vi "VIH UI - Property Page - Master Rule.vi"() -> ()   [LabVIEW 2014]
doc: "::: VI Helpeks :::\nCopyright (c) 2000-2026 Konstantin Shifershteyn. All rights reserved."
uses:
  _VIH HelpGen.llb/VIH HelpGen Typedef - Enum - Default,Enable,Disable.ctl
  _VIH HelpGen.llb/VIH HelpGen Typedef - Enum - Description Mode.ctl
  _VIH UI Controls.llb/VIH UI Control - Button - Insert HREF.ctl
  _VIH UI Controls.llb/VIH UI Control - Button - Insert Bold.ctl
  _VIH UI Controls.llb/VIH UI Control - Button - Insert Italic.ctl
  _VIH UI Controls.llb/VIH UI Control - Button - Insert Underline.ctl
  _VIH Project Manager.llb/VIH Project Tree Typedef - Tree Refnum.ctl
  VIH UI Typedef - Property Page ExtCommand.ctl
  <vilib>/Utility/miscctls.llb/LVPositionTypeDef.ctl
  <vilib>/Utility/miscctls.llb/LVPointTypeDef.ctl
  <vilib>/Utility/miscctls.llb/LVRowAndColumnUnsignedTypeDef.ctl
  <vilib>/Utility/miscctls.llb/LVSelectionTypeDef.ctl
  _VIH Support Library.llb/VIH Utility - APP - Is Value Changed (STR).vi
panel:
  out "CategoryTitle":string
  in  "%UPDATE":bool
  in  "%STOP":bool
  in  "Category List":i32(listbox)
  in  "TreeRef":T1
  in  "Tab Control":enum32{"0", "1", "2", "3", "4", "5", "6", "7"}(tab) caption="Master Rule"
  in  "PI_AddInfo":string caption="Additional Information"
  in  "PI_Email":string caption="Contact E-mail"
  in  "PI_Website":string caption="Web site"
  in  "PI_Version":string caption="Version"
  in  "PI_Copyright":string caption="Legal Copyright"
  in  "PI_Company":string caption="Company Name"
  in  "PI_Author":string caption="Author Name"
  in  "PI_Product":string caption="Product Name"
  in  "ProductInfoText":string caption="Product Info section"
  in  "ProductInfoMode":T2 caption="Product Info mode"
  out "Group Name":string
  in  "Comments":string
  in  "Dst_Image Dir":path caption="Subfolder to save image files"
  in  "Dst_HTML Dir":path caption="Subfolder to save HTML files"
  in  "Dst_JS Dir":path caption="Subfolder to save JavaScript files"
  in  "Dst_CSS Dir":path caption="Subfolder to save CSS files"
  in  "Build Root Dir":path caption="Build Root Folder"
  in  "Src_VI Template":path caption="VI Help Template File"
  in  "Src_Menu Template":path caption="Menu Help Template File"
  in  "Src_PolyVI Template":path caption="Polymorphic VI Help Template File"
  out "JS File":path caption="JS File Path"
  in  "JS List":i32[](listbox) caption="JavaScript Files"
  in  "%JS List_Add":bool caption="Add JavaScript File"
  in  "%JS List_Remove":bool caption="Remove JavaScript File"
  out "CSS File":path caption="CSS File Path"
  in  "CSS List":i32[](listbox) caption="CSS Files"
  in  "%CSS List_Add":bool caption="Add CSS File"
  in  "%CSS List_Remove":bool caption="Remove CSS File"
  in  "VIDetailsMode":T3 caption="Default VI details mode"
  in  "PVIIDscrMode":T3 caption="Default Polymorphic VI Instance description mode"
  in  "MenuItemIcons":T2 caption="Generate Palette Item Icons"
  in  "MenuDscrMode":T3 caption="Default Palette description mode"
  in  "VIDscrMode":T3 caption="Default VI description mode"
  in  "Ctl_EnumValues":T2 caption="Build list of Enum and Ring values"
  in  "Ctl_ClustMembers":T2 caption="Expand cluster members"
  in  "Ctl_DscrMode":T3 caption="VI Controls/Terminals description mode"
  in  "%CtrlRule_Insert_<I>":T4 caption="Format as Italic"
  in  "%CtrlRule_Insert_<U>":T5 caption="Format as Underline"
  in  "%CtrlRule_Insert_<B>":T6 caption="Format as Bold"
  in  "%CtrlRule_Insert_HREF":T7 caption="Insert Reference"
  in  "CtrlRule_Description":string caption="Description"
  in  "CtrlRule_CustomName":string caption="Custom Control Name"
  in  "CtrlRule_DscrMode":T3 caption="Description mode"
  in  "CtrlRule_CustomRule":bool caption="Enable custom rule"
  in  "CtrlRule_CtrlID":string caption="Control Identifier"
  in  "%CtrlRule_Edit_Enum":bool caption="Edit Enumerated Values Description"
  in  "CtrlRule_EnumValues":T2 caption="Enum and Ring values"
  in  "CtrlRule_ClustMembers":T2 caption="Cluster members"
  in  "%CtrlRule_Copy":bool caption="Copy"
  in  "%CtrlRule_Paste":bool caption="Paste"
  in  "%CtrlRule_Import":bool caption="Import VI Terminal Controls"
  in  "CtrlRule List":i32[](listbox)
  in  "%CtrlRule_Remove":bool caption="Remove"
  in  "%CtrlRule_Add":bool caption="Add"
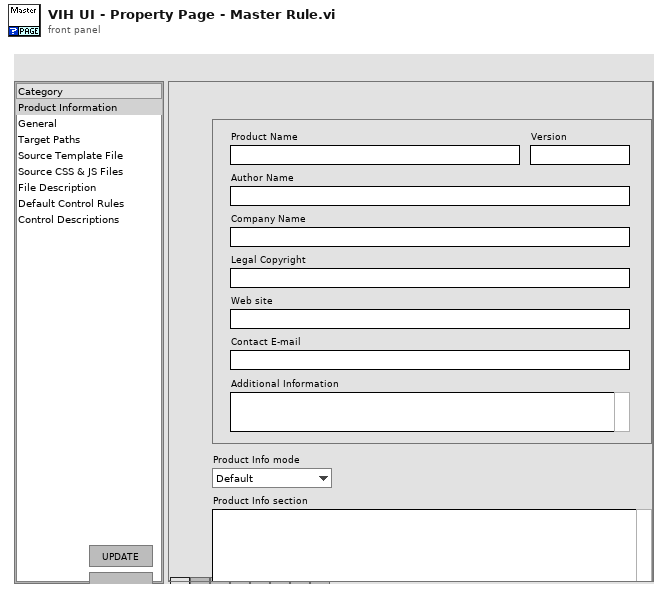
[diagram p1: front panel]
types:
  T1 = typedef "VIH Project Tree Typedef - Tree Refnum.ctl" = refnum<vi>
  T2 = typedef "VIH HelpGen Typedef - Enum - Default,Enable,Disable.ctl" = enum16{"Default", "Enable", "Disable"}
  T3 = typedef "VIH HelpGen Typedef - Enum - Description Mode.ctl" = enum16{"Default", "Description", "Description1", "Description2", "Custom", "None"}
  T4 = typedef "VIH UI Control - Button - Insert Italic.ctl" = bool
  T5 = typedef "VIH UI Control - Button - Insert Underline.ctl" = bool
  T6 = typedef "VIH UI Control - Button - Insert Bold.ctl" = bool
  T7 = typedef "VIH UI Control - Button - Insert HREF.ctl" = bool
  T8 = typedef "VIH UI Typedef - Property Page ExtCommand.ctl" = cluster{"Action":string, "Project Tree":T1, "Params":string[]}
  T9 = enum16{"Open", "Close", "Update", "Set Category"}
  T10 = enum32{"Invalid", "Standard", "Closed", "Hidden", "Minimized", "Maximized"}
  T11 = enum8{"Enabled", "Disabled", "Disabled and Grayed Out"}
  T12 = typedef "LVSelectionTypeDef.ctl" = cluster{"Selection Start":u32, "Selection End":u32}
  T13 = typedef "eventvkey.ctl" = enum16{"ASCII", "Enter", "Return", "Shift", "Ctrl", "Alt", "Cmd", "Opt", "Caps", "NumLock", "Clear", "Break", "Up", "Down", "Left", "Right", "Insert", "Delete", "Home", "End", "PageUp", "PageDown", "Escape", "Help", "Pause", "ScrollLock", "F1", "F2", "F3", "F4", "F5", "F6", "F7", "F8", "F9", "F10", "F11", "F12", "F13", "F14", "F15", "F16", "F17", "F18", "F19", "F20", "F21", "F22", "F23", "F24", "Play", "VolumeUp", "VolumeDown", "Mute", "Two Byte Char"}
  T14 = cluster{"Shift":bool, "Ctrl":bool, "Alt":bool, "Cmd":bool, "Opt":bool}
  T15 = typedef "VIH HelpGen Typedef - Cluster - Group Rule.ctl" = cluster{"Source Root Dir":path, "Build Root Dir":path, "BuildHelp":T2, "Source Paths":T16, "Target Paths":T17, "VIDscrMode":T3, "MenuDscrMode":T3, "MenuItemIcons":T2, "Control Rules":T18[], "Flags":T20, "Ctl_DscrMode":T3, "Ctl_ClustMembers":T2, "Ctl_EnumValues":T2, "%Comments":string, "PVIIDscrMode":T3, "VIDetailsMode":T3, "ProductInfoMode":T2, "ProductInfoText":string}
  T16 = typedef "VIH HelpGen Typedef - Cluster - Group Rule - Source Paths.ctl" = cluster{"CSS Files":path[], "JS Files":path[], "VI Template":path, "Menu Template":path, "PolyVI Template":path}
  T17 = typedef "VIH HelpGen Typedef - Cluster - Group Rule - Target Paths.ctl" = cluster{"HTML Dir":path, "Image Dir":path, "CSS Dir":path, "JS Dir":path}
  T18 = typedef "VIH HelpGen Typedef - Cluster - Control Rule.ctl" = cluster{"CtrlID":string, "CustomRule":bool, "DscrMode":T3, "Description":string, "ClusterMembers":T2, "EnumValues":T2, "EnumValDscr":T19[], "CustomName":string}
  T19 = typedef "VIH HelpGen Typedef - Cluster - Enum Value Info.ctl" = cluster{"Value":ext, "String":string, "Description":string}
  T20 = typedef "VIH HelpGen Typedef - Cluster - Group Rule - Flags.ctl" = cluster{"Override CSS Files":bool, "Override JS Files":bool, "Override Ctl Rules":bool}
  T21 = typedef "LVPoint32TypeDef.ctl" = cluster{"Horizontal":i32, "Vertical":i32}
  T22 = typedef "LVRowAndColumnTypeDef.ctl" = cluster{"Row":i32, "Column":i32}
  T23 = typedef "lveventtype.ctl" = enum32{"Null", "Timeout", "Annotation Menu Selection", "Annotation Menu Selection?", "App Instance Close", "App Instance Close?", "Autoscale Range Change", "Bookmark Info Change", "Cell Edit", "Cell Edit?", "Cursor Grab", "Cursor Grab?", "Cursor Menu Selection", "Cursor Menu Selection?", "Cursor Move", "Cursor Release", "Data Change", "Direction Change", "Display State Change", "Drag Ended", "Drag Enter", "Drag Leave", "Drag Over", "Drag Source Update", "Drag Starting", "Drag Starting?", "Drop", "Exec State Change", "Key Down", "Key Down?", "Key Repeat", "Key Repeat?", "Key Up", "Listbox Double Click", "Menu Activation?", "Menu Selection (App)", "Menu Selection? (App)", "Menu Selection (User)", "Mouse Down", "Mouse Down?", "Mouse Enter", "Mouse Leave", "Mouse Move", "Mouse Up", "Mouse Wheel", "NI Security User Change (App)", "Pane Size", "Panel Close", "Panel Close?", "Panel Resize", "Plot Attribute Change", "Scale Range Change", "Shortcut Menu Activation?", "Shortcut Menu Selection (App)", "Shortcut Menu Selection? (App)", "Shortcut Menu Selection (User)", "Tree Double Click", "Tree Drag", "Tree Drag?", "Tree Drop", "Tree Drop?", "Tree Item Close", "Tree Item Close?", "Tree Item Open", "Tree Item Open?", "User Event", "Value Change"}
  T24 = typedef "LVPointTypeDef.ctl" = cluster{"Horizontal":i16, "Vertical":i16}
  T25 = typedef "LVPositionTypeDef.ctl" = cluster{"Left":i32, "Top":i32}
  T26 = typedef "LVRowAndColumnUnsignedTypeDef.ctl" = cluster{"Row":u32, "Column":u32}
  T27 = typedef "VIH HelpGen Typedef - Product Info Cluster.ctl" = cluster{"ProductName":string, "Version":string, "Author":string, "Company":string, "Copyright":string, "Website":string, "Email":string, "AddInfo":string}
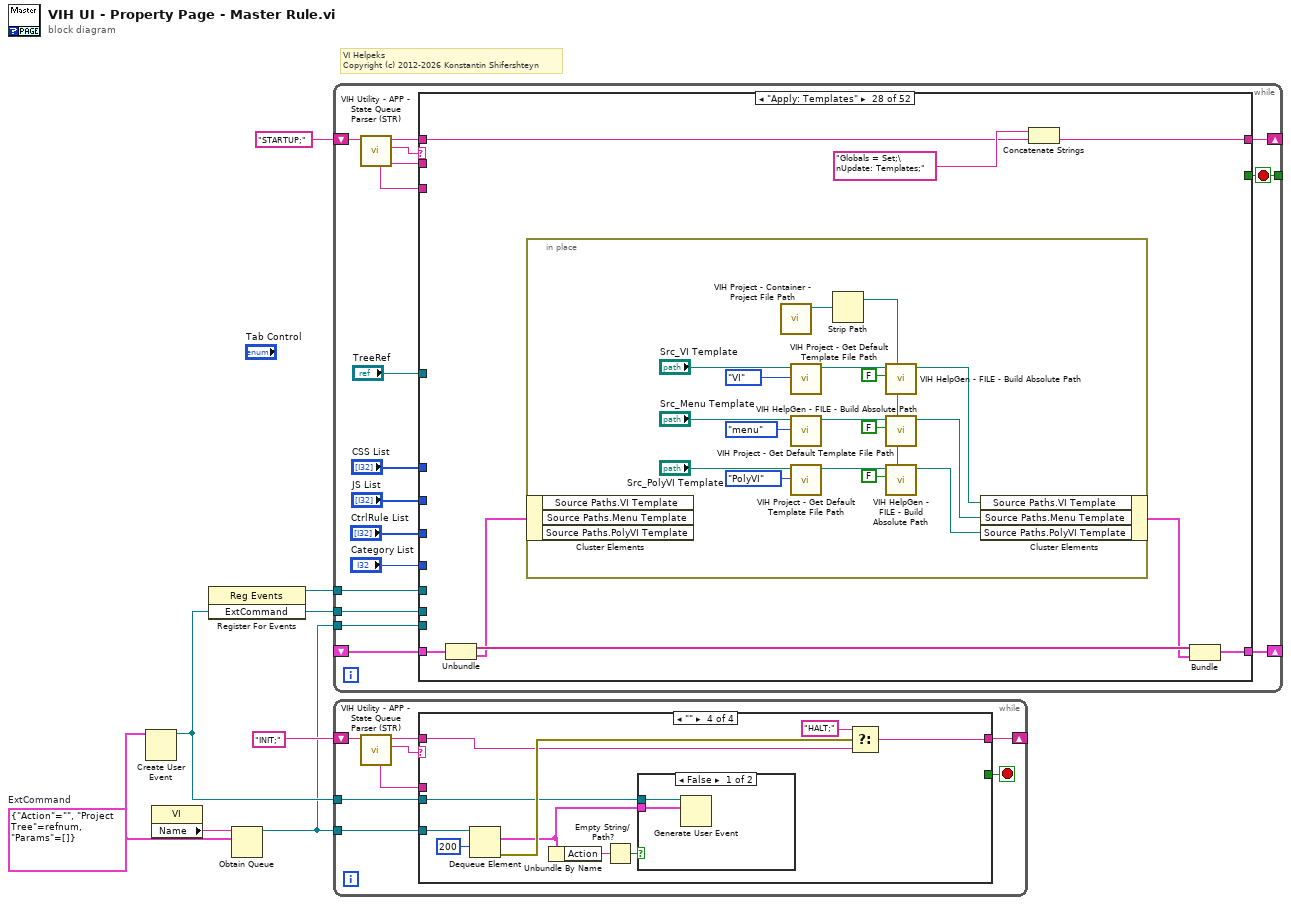
[diagram p0: block diagram]
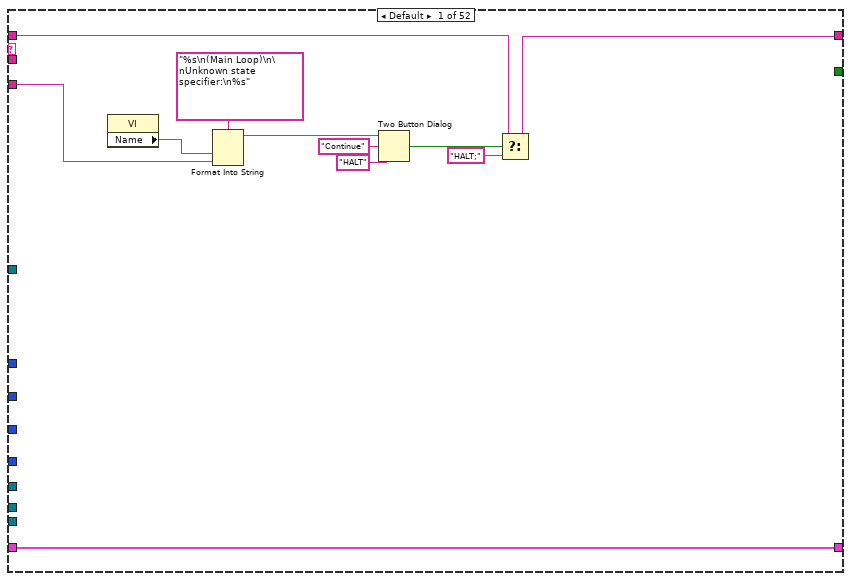
[diagram p2: hidden frame]
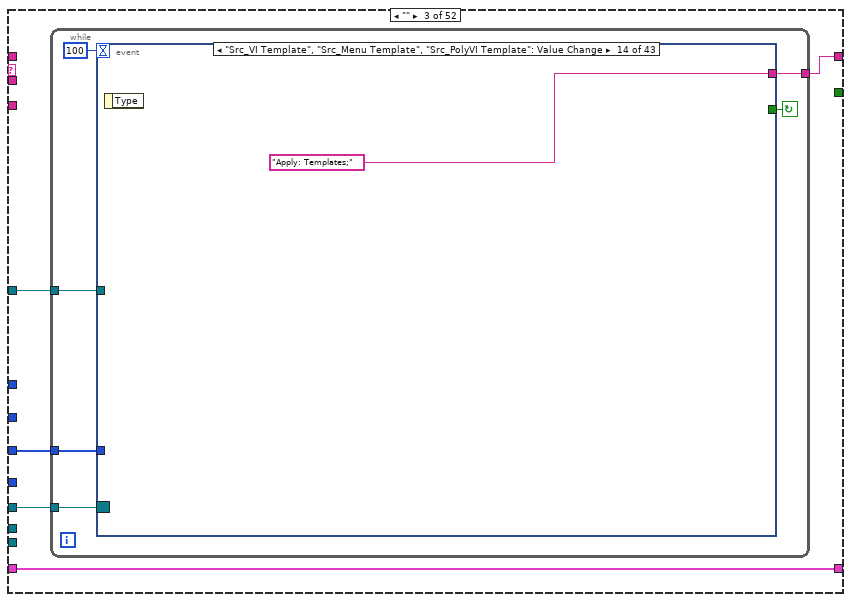
[diagram p4: hidden frame]
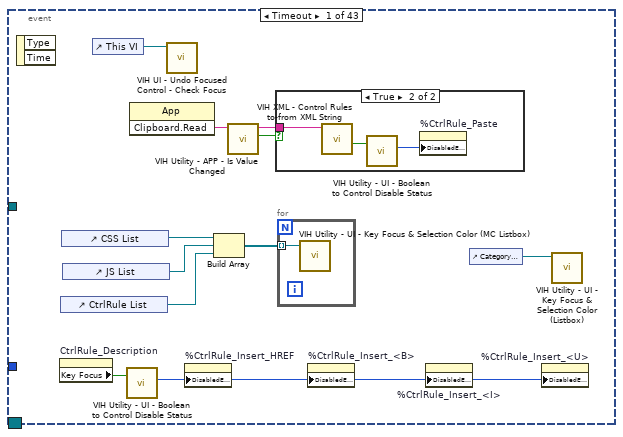
[diagram p5: hidden frame]
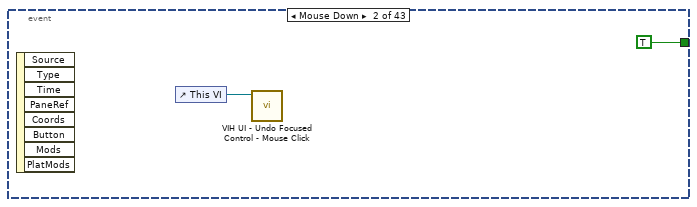
[diagram p7: hidden frame]
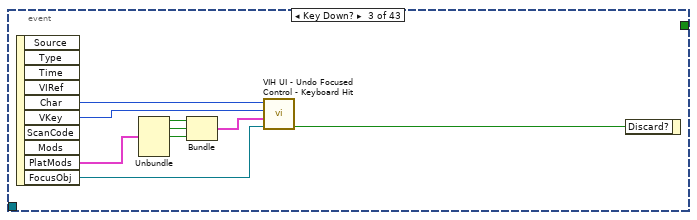
[diagram p8: hidden frame]
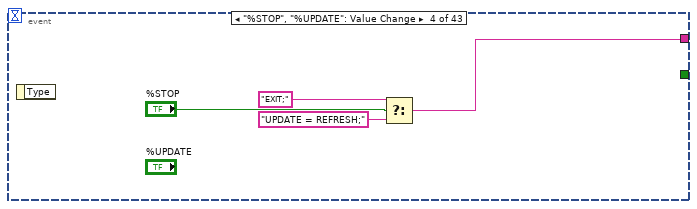
[diagram p9: hidden frame]
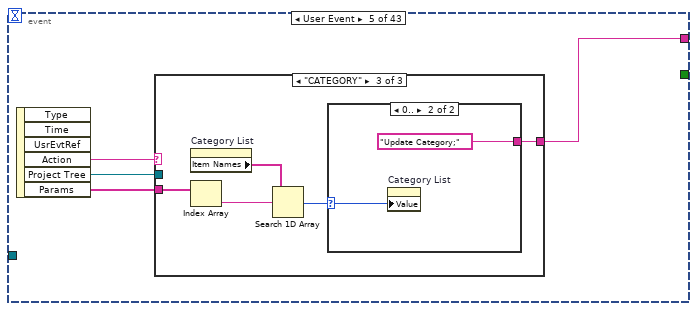
[diagram p10: hidden frame]
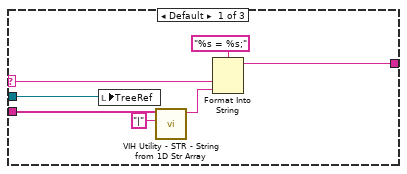
[diagram p11: hidden frame]
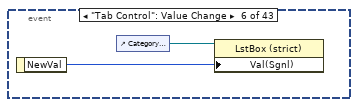
[diagram p14: hidden frame]
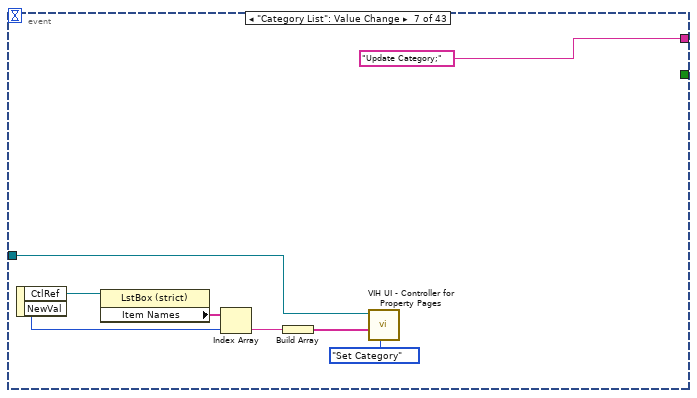
[diagram p15: hidden frame]
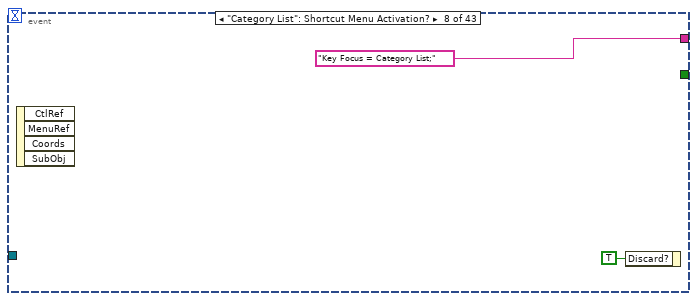
[diagram p16: hidden frame]
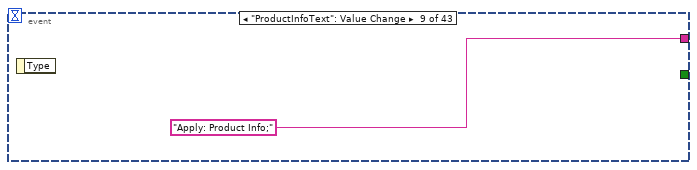
[diagram p17: hidden frame]
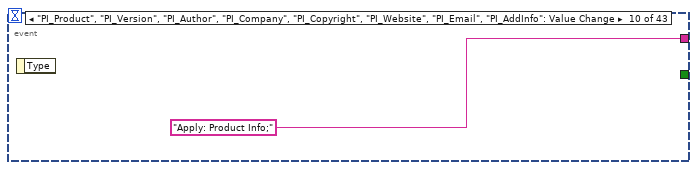
[diagram p18: hidden frame]
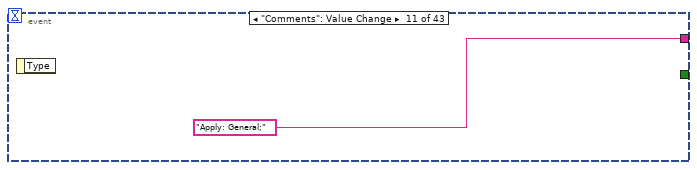
[diagram p19: hidden frame]
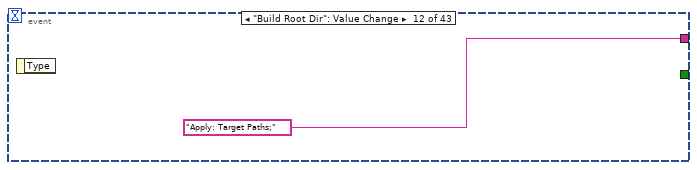
[diagram p20: hidden frame]
diagram:
  w1 = T8 {"Action"="", "Project Tree"=refnum, "Params"=[]}  # ExtCommand
  # "VI Helpeks\nCopyright (c) 2012-2026 Konstantin Shifershteyn"
  n1 = Create User Event(user event datatype=w1) -> (user event=w3:refnum<user-event>)  [unwired: 1 in, 1 out]
  n2 = property class="VI"() -> ("Name"=w6:string)  [unwired: 2 in, 2 out]
  n3 = register-events(w3) -> (reference out=w5:refnum<event-registration>)  [unwired: 2 in, 1 out]
  n4 = Obtain Queue(name (unnamed)=w6, element data type=w1) -> (queue out=w2:refnum<queue>)  [unwired: 3 in, 2 out]
  n5 = while {
    shift-right: [w21] -> _
    shift-left: "STARTUP;" -> [w24]
    tunnel: [w19] -> _
    tunnel: w5 -> [w18]
    tunnel: w3 -> [w17]
    tunnel: w2 -> [w16]
    shift-right: [w13] -> _
    shift-left: _ -> [w12]
    stop <- w19 stop-if-true
    n6 = call "VIH Utility - APP - State Queue Parser (STR).vi"("input queue"=w24) -> ("state parameters"=w15:string, "state"=w23:string, "remained queue"=w20:string, "complete state specifier"=w22:string)  [unwired: 5 in]
    n7 = case shown="\"Apply: Templates\"" w23 {
      tunnel: w22 -> [w31 _ _ _ _ _ _ _ _ w413 _ _ _ _ _ _ _ _ _ _ _ _ _ _ _ _ _ _ _ _ _ _ _ _ _ _ _ _ _ _ _ _ _ _ _ _ _ _ _ _ _ _]
      tunnel: [w26 w36 w41 "INIT;\nUPDATE;" w349 "HALT;" w379 w382 w405 w415 w437 w440 w444 w460 w467 w486 w492 w514 w547 w563 w583 w598 w610 w624 w637 w647 w656 w669 w694 w711 w729 w759 w785 w835 w844 w866 w882 w918 w938 w962 w971 w980 w992 w1018 w1042 w1057 w1066 w1075 w1087 w1113 w1137 w1152] -> w21
      tunnel: w20 -> [w27 w36 _ _ w349 _ w379 w382 w406 w415 w437 w440 w444 w460 w467 w486 w492 w514 w547 w563 w583 w598 w610 w624 w643 w653 w657 w670 w695 w711 w729 w764 w786 w835 w847 w871 w889 w923 w945 w962 w971 w980 w996 w1023 w1047 w1057 w1066 w1075 w1091 w1118 w1142 w1152]
      tunnel: [_ _ _ _ _ _ TRUE _ _ _ _ _ _ _ _ _ _ _ _ _ _ _ _ _ _ _ _ _ _ _ _ _ _ _ _ _ _ _ _ _ _ _ _ _ _ _ _ _ _ _ _ _] -> w19
      tunnel: w18 -> [_ _ w42 _ _ _ w378 _ _ _ _ _ _ _ _ _ _ _ _ _ _ _ _ _ _ _ _ _ _ _ _ _ _ _ _ _ _ _ _ _ _ _ _ _ _ _ _ _ _ _ _ _]
      tunnel: w17 -> [_ _ _ _ _ _ w377 _ _ _ _ _ _ _ _ _ _ _ _ _ _ _ _ _ _ _ _ _ _ _ _ _ _ _ _ _ _ _ _ _ _ _ _ _ _ _ _ _ _ _ _ _]
      tunnel: w16 -> [_ _ _ _ _ _ w375 _ _ _ _ _ _ _ _ _ _ _ _ _ _ _ _ _ _ _ _ _ _ _ _ _ _ _ _ _ _ _ _ _ _ _ _ _ _ _ _ _ _ _ _ _]
      tunnel: w15 -> [_ _ _ _ _ _ _ _ w394 w414 _ w438 w442 _ _ _ _ _ _ _ _ _ _ _ _ _ _ _ _ _ w712 _ w781 _ _ _ w880 w909 w936 _ _ _ _ _ _ _ _ _ _ _ _ _]
      tunnel: "Category List" -> [_ _ _ _ _ _ _ _ _ _ w435 _ _ _ _ _ _ _ _ _ _ _ _ _ _ _ _ _ _ _ _ _ _ _ _ _ _ _ _ _ _ _ _ _ _ _ _ _ _ _ _ _]
      tunnel: [w25 w37 w40 w307 w348 w360 w373 w381 w402 w417 w434 w439 w443 w459 w462 w483 w491 w513 w546 w562 w582 w597 w609 w623 w640 w650 w661 w674 w699 w710 w728 w760 w784 w829 w845 w867 w884 w919 w940 w961 w968 w979 w993 w1019 w1043 w1056 w1063 w1074 w1088 w1114 w1138 w1151] -> w13
      tunnel: w12 -> [w25 w37 w40 w307 w348 w360 w373 w381 w401 w416 w434 w439 w443 w459 w462 w483 w491 w513 w546 w562 w582 w597 w609 w623 w642 w652 w663 w676 w701 w710 w728 w761 w787 w829 w846 w868 w885 w920 w941 w961 w968 w979 w994 w1020 w1044 w1056 w1063 w1074 w1089 w1115 w1139 w1151]
      tunnel: "CtrlRule List" -> [_ _ w39 _ _ _ _ _ _ _ _ _ _ _ _ _ _ _ _ _ _ _ w600 _ _ _ _ _ _ _ w718 w752 w779 w827 w840 _ _ _ _ _ _ _ _ _ _ _ _ _ _ _ _ _]
      tunnel: "CSS List" -> [_ _ _ _ _ _ _ _ _ _ _ _ _ _ _ _ _ _ _ w553 _ _ _ _ _ _ _ _ _ _ _ _ _ _ _ _ _ _ _ _ w965 _ w984 w1016 _ _ _ _ _ _ _ _]
      tunnel: "JS List" -> [_ _ _ _ _ _ _ _ _ _ _ _ _ _ _ _ _ _ _ _ w573 _ _ _ _ _ _ _ _ _ _ _ _ _ _ _ _ _ _ _ _ _ _ _ _ _ w1058 _ w1077 w1111 _ _]
      tunnel: "TreeRef" -> [_ _ w38 _ _ _ _ _ _ _ _ _ _ _ w463 _ _ _ _ _ _ _ _ _ _ _ _ _ _ _ _ _ w777 _ _ _ _ _ w935 _ _ _ _ _ _ _ _ _ _ _ _ _]
      frame Default {
        n8 = property class="VI"() -> ("Name"=w30:string)  [unwired: 2 in, 2 out]
        n9 = Format Into String(format string="%s\n(Main Loop)\n\nUnknown state specifier:\n%s", w30, w31) -> (resulting string=w34:string)  [unwired: 2 in, 1 out]
        n10 = Two Button Dialog(message=w34, 1:"HALT" ("F button name (\"Cancel\")"), 2:"Continue" ("T button name (\"OK\")")) -> (T button?=w28:bool)
        n11 = Select(t=w27, s=w28, f="HALT;") -> (s? t:f=w26:string)
      }
      frame "#" {
      }
      frame "" {
        n12 = while {
          tunnel: w42 -> [w47]
          tunnel: [w46] -> w41
          tunnel: w39 -> [w45]
          tunnel: w38 -> [w44]
          stop <- w43 continue-if-true
          n13 = event shown="[13] \"Src_VI Template\", \"Src_Menu Template\", \"Src_PolyVI Template\": Value Change" {
            selector: w47 -> [_ _ _ _ _ _ _ _ _ _ _ _ _ _ _ _ _ _ _ _ _ _ _ _ _ _ _ _ _ _ _ _ _ _ _ _ _ _ _ _ _ _ _]
            dyn-events: _ -> [_ _ _ _ _ _ _ _ _ _ _ _ _ _ _ _ _ _ _ _ _ _ _ _ _ _ _ _ _ _ _ _ _ _ _ _ _ _ _ _ _ _ _]
            timeout: 100 -> [_ _ _ _ _ _ _ _ _ _ _ _ _ _ _ _ _ _ _ _ _ _ _ _ _ _ _ _ _ _ _ _ _ _ _ _ _ _ _ _ _ _ _]
            tunnel: [_ _ _ w76 w82 _ "Update Category;" ("string") "Key Focus = Category List;" ("string") "Apply: Product Info;" ("string") "Apply: Product Info;" ("string") "Apply: General;" ("string") "Apply: Target Paths;" ("string") "Apply: Target Paths;" ("string") "Apply: Templates;" ("string") "Apply: Item Rules;" ("string") "Apply: Item Rules;" ("string") "CtrlRule: Update Controls = INIT;" ("string") w137 w145 w160 w175 "Key Focus = CtrlRule List;" ("output string") w180 w186 w202 w203 "CSS List: Update Controls;" w214 "Key Focus = CSS List;" ("output string") w218 "JS List: Update Controls;" w227 "Key Focus = JS List;" ("output string") w231 _ _ _ _ _ _ _ _ _] -> w46
            tunnel: w45 -> [_ _ _ _ _ _ _ _ _ _ _ _ _ _ _ _ _ _ w142 _ _ _ _ _ w195 w204 _ _ _ _ _ _ _ _ _ _ _ _ _ _ _ _ _]
            tunnel: w44 -> [_ _ _ _ _ _ w99 _ _ _ _ _ _ _ _ _ _ _ _ _ _ _ _ _ _ _ _ _ _ _ _ _ _ _ w250 w251 w257 w260 w266 w269 w275 w278 w284]
            tunnel: [_ TRUE _ _ _ _ _ _ _ _ _ _ _ _ _ _ _ _ _ _ _ _ _ _ _ _ _ _ _ _ _ _ _ _ _ _ _ _ _ _ _ _ _] -> w43
            event Timeout {
              n14 = event-data() -> ()  [unwired: 1 in, 2 out]
              n15 = property on="CtrlRule_Description" class="Str"() -> ("Key Focus"=w51:bool)  [unwired: 2 in, 2 out]
              n16 = control-ref of="CtrlRule List"() -> (w57:refnum<vi>)
              n17 = control-ref of="CSS List"() -> (w59:refnum<vi>)
              n18 = control-ref of="JS List"() -> (w58:refnum<vi>)
              n19 = control-ref of="This VI"() -> (w49:refnum<vi>)
              n20 = call "VIH Utility - UI - Boolean to Control Disable Status.vi"("Status in"=w51) -> ("Control Disable if False"=w50:u8)  [unwired: 3 in, 1 out]
              n21 = invoke class="App" method="Clipboard.Read"() -> ("Read Clipbrd"=w52:string)  [unwired: 3 in, 2 out]
              n22 = call "VIH UI - Undo Focused Control - Check Focus.vi"("VI Refnum"=w49) -> ()  [unwired: 10 in, 1 out]
              n23 = property on="%CtrlRule_Insert_HREF" class="Bool"("DisabledEnum"=w50) -> ()  [unwired: 2 in, 2 out]
              n24 = Build Array(w59, w58, w57) -> (w56:refnum<vi>[])
              n25 = call-poly "VIH Utility - APP - Is Value Changed.vi"("Value"=w52) -> ("Changed"=w54:bool, "dup Value"=w53:string)  [unwired: 5 in]
              n26 = case shown="True" w54 {
                tunnel: w53 -> [_ w60]
                frame False {
                }
                frame True {
                  n27 = call "VIH XML - Control Rules to-from XML String.vi"("XML in"=w60) -> ("available"=w62:bool)  [unwired: 7 in, 3 out]
                  n28 = call "VIH Utility - UI - Boolean to Control Disable Status.vi"("Status in"=w62) -> ("Control Disable if False"=w61:u8)  [unwired: 3 in, 1 out]
                  n29 = property on="%CtrlRule_Paste" class="Bool"("DisabledEnum"=w61) -> ()  [unwired: 2 in, 2 out]
                }
              }
              n30 = for {
                tunnel: w56 -> [w63] mode=indexing
                n31 = call "VIH Utility - UI - Key Focus & Selection Color (MC Listbox).vi"("MCListbox Refnum"=w63) -> ()  [unwired: 8 in, 3 out]
              }
              n32 = property on="%CtrlRule_Insert_<B>" class="Bool"("DisabledEnum"=w50) -> ()  [unwired: 2 in, 2 out]
              n33 = property on="%CtrlRule_Insert_<I>" class="Bool"("DisabledEnum"=w50) -> ()  [unwired: 2 in, 2 out]
              n34 = control-ref of="Category List"() -> (w55:refnum<vi>)
              n35 = property on="%CtrlRule_Insert_<U>" class="Bool"("DisabledEnum"=w50) -> ()  [unwired: 2 in, 2 out]
              n36 = call "VIH Utility - UI - Key Focus & Selection Color (Listbox).vi"("LstBox Refnum"=w55) -> ()  [unwired: 8 in, 3 out]
            }
            event Mouse Down {
              n37 = event-data() -> ()  [unwired: 1 in, 8 out]
              n38 = control-ref of="This VI"() -> (w65:refnum<vi>)
              n39 = call "VIH UI - Undo Focused Control - Mouse Click.vi"("VI Refnum"=w65) -> ()  [unwired: 9 in, 2 out]
            }
            event Key Down? {
              n40 = event-data() -> ("Char"=w74:i16, "VKey"=w73:T13, "PlatMods"=w72:T14, "FocusObj"=w67:refnum<vi>)  [unwired: 1 in, 6 out]
              n41 = Unbundle(w72) -> ("Shift"=w71:bool, "Ctrl"=w70:bool, "Alt"=w69:bool)  [unwired: 2 out]
              n42 = Bundle("Shift"=w71, "Ctrl"=w70, "Alt"=w69) -> (w68:cluster{"Shift":bool, "Ctrl":bool, "Alt":bool})  [unwired: 1 in]
              n43 = call "VIH UI - Undo Focused Control - Keyboard Hit.vi"("FocusObj"=w67, "PlatMods"=w68, "VKey"=w73, "Char"=w74) -> ("Discard"=w66:bool)  [unwired: 7 in]
              n44 = event-data("Discard?"=w66) -> ()  [unwired: 1 in, 1 out]
            }
            event "%STOP", "%UPDATE": Value Change {
              n45 = event-data() -> ()  [unwired: 1 in, 1 out]
              n46 = Select(t="EXIT;", s="%STOP", f="UPDATE = REFRESH;") -> (s? t:f=w76:string)
            }
            event User Event {
              n47 = event-data() -> ("Action"=w79:string, "Project Tree"=w80:T1, "Params"=w81:string[])  [unwired: 1 in, 3 out]
              n48 = case shown="\"CATEGORY\"" w79 {
                selector: w79 -> [w83 _ _]
                tunnel: w81 -> [w89 _ w93]
                tunnel: [w85 _ w90] -> w82
                tunnel: w80 -> [w84 _ _]
                frame Default {
                  n49 = local write "TreeRef"(w84) -> ()
                  n50 = call "VIH Utility - STR - String from 1D Str Array.vi"("delimiter ('\\n')"="|" ("delimiter ('\\n')"), "Array in"=w89) -> ("String out"=w86:string)  [unwired: 5 in]
                  n51 = Format Into String(format string="%s = %s;", w83, w86) -> (resulting string=w85:string)  [unwired: 2 in, 1 out]
                }
                frame "" {
                }
                frame "CATEGORY" {
                  n52 = property on="Category List" class="LstBox (strict)"() -> ("Item Names"=w92:string[])  [unwired: 2 in, 2 out]
                  n53 = Index Array(array=w93) -> (element=w94:string)  [unwired: 1 in]
                  n54 = Search 1D Array(1D array=w92, element=w94) -> (index of element=w91:i32)  [unwired: 1 in]
                  n55 = case shown="0.." w91 {
                    selector: w91 -> [_ w96]
                    tunnel: [_ "Update Category;" ("string")] -> w90
                    frame ..-1 {
                    }
                    frame 0.. {
                      n56 = property on="Category List" class="LstBox (strict)"("Value"=w96) -> ()  [unwired: 2 in, 2 out]
                    }
                  }
                }
              }
            }
            event "Tab Control": Value Change {
              n57 = event-data() -> ("NewVal"=w97:enum32{"0", "1", "2", "3", "4", "5", "6", "7"})  [unwired: 1 in]
              n58 = control-ref of="Category List"() -> (w98:refnum<vi>)
              n59 = property class="LstBox (strict)"(reference=w98, "Val(Sgnl)"=w97) -> ()  [unwired: 1 in, 2 out]
            }
            event "Category List": Value Change {
              n60 = event-data() -> ("CtlRef"=w104:refnum<vi>, "NewVal"=w103:i32)  [unwired: 1 in]
              n61 = property class="LstBox (strict)"(reference=w104) -> ("Item Names"=w105:string[])  [unwired: 1 in, 2 out]
              n62 = Index Array(array=w105, index=w103) -> (element=w101:string)
              n63 = Build Array(w101) -> (w100:string[])
              n64 = call "VIH UI - Controller for Property Pages.vi"("cmd (update)"=T9."Set Category", "Params"=w100, "Project Tree"=w99) -> ()  [unwired: 7 in, 2 out]
            }
            event "Category List": Shortcut Menu Activation? {
              n65 = event-data() -> ()  [unwired: 1 in, 4 out]
              n66 = event-data("Discard?"=TRUE) -> ()  [unwired: 1 in, 1 out]
            }
            event "ProductInfoText": Value Change {
              n67 = event-data() -> ()  [unwired: 1 in, 1 out]
            }
            event "PI_Product", "PI_Version", "PI_Author", "PI_Company", "PI_Copyright", "PI_Website", "PI_Email", "PI_AddInfo": Value Change {
              n68 = event-data() -> ()  [unwired: 1 in, 1 out]
            }
            event "Comments": Value Change {
              n69 = event-data() -> ()  [unwired: 1 in, 1 out]
            }
            event "Build Root Dir": Value Change {
              n70 = event-data() -> ()  [unwired: 1 in, 1 out]
            }
            event "Dst_HTML Dir", "Dst_Image Dir", "Dst_CSS Dir", "Dst_JS Dir": Value Change {
              n71 = event-data() -> ("CtlRef"=w114:refnum<vi>, "NewVal"=w113:path)  [unwired: 1 in]
              n72 = Empty String/Path?(string/path=w113) -> (empty?=w115:bool)
              n73 = case shown="False" w115 {
                tunnel: w114 -> [w119 _]
                tunnel: w113 -> [w117 _]
                frame False {
                  n74 = Path Type(1:w117) -> (0:w118:i16)
                  n75 = case shown="0" w118 {
                    tunnel: w119 -> [w124 _ w126]
                    tunnel: w117 -> [w122 _ _]
                    frame 0 {
                      # "If absolute path was enered"
                      n76 = call "VIH Project - Container - Master Rule.vi"() -> ("Rule out"=w123:T15)  [unwired: 11 in]
                      n77 = Unbundle By Name(w123) -> ("Build Root Dir"=w120:path)
                      n78 = call "VIH HelpGen - FILE - Build Relative Path.vi"("Root Path"=w120, "Path in"=w122) -> ("Path out"=w121:path)  [unwired: 9 in]
                      n79 = property class="Path"(reference=w124, "Value"=w121) -> ()  [unwired: 1 in, 2 out]
                    }
                    frame 1 {
                    }
                    frame 2, Default {
                      # "Not A Path"
                      n80 = property class="Path"(reference=w126, "Value"=path "") -> ()  [unwired: 1 in, 2 out]
                    }
                  }
                }
                frame True {
                }
              }
            }
            event "Src_VI Template", "Src_Menu Template", "Src_PolyVI Template": Value Change {
              n81 = event-data() -> ()  [unwired: 1 in, 1 out]
            }
            event Value Change {
              n82 = event-data() -> ()  [unwired: 1 in, 1 out]
            }
            event Value Change {
              n83 = event-data() -> ()  [unwired: 1 in, 1 out]
            }
            event "CtrlRule List": Value Change {
              n84 = event-data() -> ()  [unwired: 1 in, 1 out]
            }
            event "CtrlRule List": Double Click {
              n85 = event-data() -> ("CtlRef"=w136:refnum<vi>, "Row"=w134:i32)  [unwired: 1 in, 6 out]
              n86 = property class="MCListbox (strict)"(reference=w136) -> ("ItemNames"=w135:string[][])  [unwired: 1 in, 2 out]
              n87 = Index Array(array=w135, index (row)=w134, index (col)=1 ("disabled index (col)")) -> (element=w132:string)
              n88 = Empty String/Path?(string/path=w132) -> (empty?=w131:bool)
              n89 = case shown="False" w131 {
                tunnel: [w140 _] -> w137
                tunnel: w134 -> [w138 _]
                frame False {
                  n90 = Format Into String(format string="CtrlRule: Edit Enum Values = %d;" ("string"), w138) -> (resulting string=w140:string)  [unwired: 2 in, 1 out]
                }
                frame True {
                }
              }
            }
            event "CtrlRule List": Edit Cell {
              n91 = event-data() -> ("String"=w143:string)  [unwired: 1 in, 4 out]
              n92 = Index Array(array=w142) -> (element=w141:i32)  [unwired: 1 in]
              n93 = local write "CtrlRule_CtrlID"(w143) -> ()
              n94 = Format Into String(format string="CtrlRule: Apply = %d;" ("string"), w141) -> (resulting string=w145:string)  [unwired: 2 in, 1 out]
            }
            event "CtrlRule List": Mouse Up {
              n95 = event-data() -> ("CtlRef"=w157:refnum<vi>, "Coords"=w159:T21, "Button"=w158:u16)  [unwired: 1 in, 2 out]
              n96 = property class="MCListbox (strict)"(reference=w157) -> ("ItemSyms"=w147:i32[])  [unwired: 1 in, 2 out]
              n97 = invoke class="MCListbox (strict)" method="Point To Row Column"(reference=w157, "Point"=w159) -> ("CellPosition"=w155:T22, "InGlyph"=w150:bool)  [unwired: 5 in, 5 out]
              n98 = Equal?(x=w158, y=u16 1) -> (x = y?=w151:bool)
              n99 = Array Size(array=w147) -> (size(s)=w154:i32)
              n100 = Unbundle By Name(w155) -> ("Row"=w153:i32)
              n101 = In Range and Coerce(upper limit=w154, x=w153, lower limit=0) -> (coerced(x)=w146:i32, In Range?=w149:bool)
              n102 = Compound Arithmetic op=AND(w150, w151, w149) -> (w148:bool)
              n103 = case shown="True" w148 {
                tunnel: [_ w162] -> w160
                tunnel: w147 -> [_ w173]
                tunnel: w146 -> [_ w163]
                frame False {
                }
                frame True {
                  n104 = Index Array(array=w173, index=w163) -> (element=w171:i32)
                  n105 = Build Array(w163) -> (w165:i32[])
                  n106 = And(x=65535, y=w171) -> (x .and. y?=w170:i32)
                  n107 = Equal?(x=w170, y=37) -> (x = y?=w161:bool)
                  n108 = Number To Decimal String(number=w165) -> (decimal integer string=w164:string[])  [unwired: 1 in]
                  n109 = call "VIH Utility - STR - String from 1D Str Array.vi"("delimiter ('\\n')"="," ("delimiter ('\\n')"), "Array in"=w164) -> ("String out"=w166:string)  [unwired: 5 in]
                  n110 = Format Into String(format string="CtrlRule: Enable = %d ? %s;" ("string"), w161, w166) -> (resulting string=w162:string)  [unwired: 2 in, 1 out]
                }
              }
            }
            event "CtrlRule List": Drag Ended {
              n111 = event-data() -> ("Result"=w174:enum16{"Drop Cancel", "Drop Move", "Drop Copy"})  [unwired: 1 in, 1 out]
              n112 = case shown="\"Drop Move\"" w174 {
                tunnel: [_ "CtrlRule: Dragged;"] -> w175
                frame Default {
                }
                frame "Drop Move" {
                }
              }
            }
            event "CtrlRule List": Shortcut Menu Activation? {
              n113 = event-data() -> ()  [unwired: 1 in, 4 out]
              n114 = event-data("Discard?"=TRUE) -> ()  [unwired: 1 in, 1 out]
            }
            event "%CtrlRule_Add", "%CtrlRule_Remove": Value Change {
              n115 = event-data() -> ()  [unwired: 1 in, 1 out]
              n116 = Build Array("%CtrlRule_Add", "%CtrlRule_Remove") -> (w183:bool[])
              n117 = Search 1D Array(1D array=w183, element=TRUE) -> (index of element=w181:i32)  [unwired: 1 in]
              n118 = Pick Line(multi-line string="CtrlRule: Add;              Key Focus = CtrlRule Control Name;\nCtrlRule: Remove;       Key Focus = CtrlRule List;" ("string"), line index=w181) -> (output string=w180:string)  [unwired: 1 in]
            }
            event "%CtrlRule_Import", "%CtrlRule_Paste", "%CtrlRule_Copy": Value Change {
              n119 = event-data() -> ()  [unwired: 1 in, 1 out]
              n120 = Build Array("%CtrlRule_Import", "%CtrlRule_Paste", "%CtrlRule_Copy") -> (w190:bool[])
              n121 = Search 1D Array(1D array=w190, element=TRUE) -> (index of element=w192:i32)  [unwired: 1 in]
              n122 = Pick Line(multi-line string="CtrlRule: Import = VI;    Key Focus = CtrlRule List;\nCtrlRule: Import = CB;   Key Focus = CtrlRule List;\nCtrlRule: Export = CB;   Key Focus = CtrlRule List;" ("string"), line index=w192) -> (output string=w186:string)  [unwired: 1 in]
            }
            event "CtrlRule_CtrlID", "CtrlRule_CustomRule", "CtrlRule_Description", "CtrlRule_CustomName": Value Change {
              n123 = event-data() -> ()  [unwired: 1 in, 1 out]
              n124 = Index Array(array=w195) -> (element=w197:i32)  [unwired: 1 in]
              n125 = Array Size(array=w195) -> (size(s)=w200:i32)
              n126 = Equal?(x=w200, y=1) -> (x = y?=w198:bool)
              n127 = Select(t=w197, s=w198, f=-1) -> (s? t:f=w194:i32)
              n128 = Format Into String(format string="CtrlRule: Apply = %d;" ("string"), w194) -> (resulting string=w202:string)  [unwired: 2 in, 1 out]
            }
            event "%CtrlRule_Edit_Enum": Value Change {
              n129 = event-data() -> ()  [unwired: 1 in, 1 out]
              n130 = Index Array(array=w204) -> (element=w206:i32)  [unwired: 1 in]
              n131 = Array Size(array=w204) -> (size(s)=w208:i32)
              n132 = Equal?(x=w208, y=1) -> (x = y?=w205:bool)
              n133 = case shown="True" w205 {
                tunnel: [_ w211] -> w203
                tunnel: w206 -> [_ w209]
                frame False {
                }
                frame True {
                  n134 = Format Into String(format string="CtrlRule: Edit Enum Values = %d;" ("string"), w209) -> (resulting string=w211:string)  [unwired: 2 in, 1 out]
                }
              }
            }
            event "CSS List": Value Change {
              n135 = event-data() -> ()  [unwired: 1 in, 1 out]
            }
            event "CSS List": Drag Ended {
              n136 = event-data() -> ("Result"=w213:enum16{"Drop Cancel", "Drop Move", "Drop Copy"})  [unwired: 1 in, 1 out]
              n137 = case shown="\"Drop Move\"" w213 {
                tunnel: [_ "CSS List: Dragged;"] -> w214
                frame Default {
                }
                frame "Drop Move" {
                }
              }
            }
            event "CSS List": Shortcut Menu Activation? {
              n138 = event-data() -> ()  [unwired: 1 in, 1 out]
              n139 = event-data("Discard?"=TRUE) -> ()  [unwired: 1 in, 1 out]
            }
            event "%CSS List_Add", "%CSS List_Remove": Value Change {
              n140 = event-data() -> ()  [unwired: 1 in, 1 out]
              n141 = Build Array("%CSS List_Add", "%CSS List_Remove") -> (w224:bool[])
              n142 = Search 1D Array(1D array=w224, element=TRUE) -> (index of element=w222:i32)  [unwired: 1 in]
              n143 = Pick Line(multi-line string="CSS List: Add;         Key Focus = CSS List;\nCSS List: Remove;  Key Focus = CSS List;", line index=w222) -> (output string=w218:string)  [unwired: 1 in]
            }
            event "JS List": Value Change {
              n144 = event-data() -> ()  [unwired: 1 in, 1 out]
            }
            event "JS List": Drag Ended {
              n145 = event-data() -> ("Result"=w226:enum16{"Drop Cancel", "Drop Move", "Drop Copy"})  [unwired: 1 in, 1 out]
              n146 = case shown="\"Drop Move\"" w226 {
                tunnel: [_ "JS List: Dragged;"] -> w227
                frame Default {
                }
                frame "Drop Move" {
                }
              }
            }
            event "JS List": Shortcut Menu Activation? {
              n147 = event-data() -> ()  [unwired: 1 in, 4 out]
              n148 = event-data("Discard?"=TRUE) -> ()  [unwired: 1 in, 1 out]
            }
            event "%JS List_Add", "%JS List_Remove": Value Change {
              n149 = event-data() -> ()  [unwired: 1 in, 1 out]
              n150 = Build Array("%JS List_Add", "%JS List_Remove") -> (w237:bool[])
              n151 = Search 1D Array(1D array=w237, element=TRUE) -> (index of element=w235:i32)  [unwired: 1 in]
              n152 = Pick Line(multi-line string="JS List: Add;         Key Focus = JS List;\nJS List: Remove;  Key Focus = JS List;", line index=w235) -> (output string=w231:string)  [unwired: 1 in]
            }
            event Value Change {
              n153 = event-data() -> ()  [unwired: 1 in, 1 out]
              n154 = control-ref of="CtrlRule_Description"() -> (w249:refnum<vi>)
              n155 = Build Array("%CtrlRule_Insert_HREF", "%CtrlRule_Insert_<B>", "%CtrlRule_Insert_<I>", "%CtrlRule_Insert_<U>") -> (w248:T5[])
              n156 = Search 1D Array(1D array=w248, element=TRUE) -> (index of element=w242:i32)  [unwired: 1 in]
              n157 = Increment(x=w242) -> (x+1=w241:i32)
              n158 = Type Cast(type=enum32{"nop", "<a>", "<b>", "<i>", "<u>"}."nop" ("cmd"), x=w241) -> (*(type *) &x=w239:enum32{"nop", "<a>", "<b>", "<i>", "<u>"})
              n159 = call "VIH UI - Insert HTML Tag to String.vi"("cmd"=w239, "Project Tree"=w250, "Str Refnum"=w249) -> ("dup Str Refnum"=w238:refnum<vi>)  [unwired: 8 in]
              n160 = call "VIH UI - Undo Focused Control - Core.vi"("Ctl Refnum"=w238) -> ()  [unwired: 8 in, 3 out]
            }
            event "ProductInfoText": Shortcut Menu Activation? {
              n161 = event-data() -> ("Type"=w254:T23, "CtlRef"=w253:refnum<vi>, "MenuRef"=w252:refnum<k9>)  [unwired: 1 in, 1 out]
              n162 = call "VIH UI - String Shortcut Menu Handler.vi"("Project Tree"=w251, "mode"=enum16{"basic", "format 1", "format 2"}."format 2", "menu"=w252, "Str Refnum"=w253, "Type"=w254) -> ()  [unwired: 7 in]
              n163 = event-data() -> ()  [unwired: 2 in, 1 out]
            }
            event "ProductInfoText": Shortcut Menu Selection (User) {
              n164 = event-data() -> ("Type"=w259:T23, "CtlRef"=w258:refnum<vi>, "ItemTag"=w256:string)  [unwired: 1 in, 1 out]
              n165 = call "VIH UI - String Shortcut Menu Handler.vi"("Project Tree"=w257, "Menu tag"=w256, "Str Refnum"=w258, "Type"=w259) -> ()  [unwired: 8 in]
            }
            event "PI_Product", "PI_Version", "PI_Author", "PI_Company", "PI_Copyright", "PI_Website", "PI_Email", "PI_AddInfo": Shortcut Menu Activation? {
              n166 = event-data() -> ("Type"=w263:T23, "CtlRef"=w262:refnum<vi>, "MenuRef"=w261:refnum<k9>)  [unwired: 1 in, 1 out]
              n167 = call "VIH UI - String Shortcut Menu Handler.vi"("Project Tree"=w260, "mode"=enum16{"basic", "format 1", "format 2"}."basic", "menu"=w261, "Str Refnum"=w262, "Type"=w263) -> ()  [unwired: 7 in]
              n168 = event-data() -> ()  [unwired: 2 in, 1 out]
            }
            event "PI_Product", "PI_Version", "PI_Author", "PI_Company", "PI_Copyright", "PI_Website", "PI_Email", "PI_AddInfo": Shortcut Menu Selection (User) {
              n169 = event-data() -> ("Type"=w268:T23, "CtlRef"=w267:refnum<vi>, "ItemTag"=w265:string)  [unwired: 1 in, 1 out]
              n170 = call "VIH UI - String Shortcut Menu Handler.vi"("Project Tree"=w266, "Menu tag"=w265, "Str Refnum"=w267, "Type"=w268) -> ()  [unwired: 8 in]
            }
            event "CtrlRule_Description": Shortcut Menu Activation? {
              n171 = event-data() -> ("Type"=w272:T23, "CtlRef"=w271:refnum<vi>, "MenuRef"=w270:refnum<k9>)  [unwired: 1 in, 1 out]
              n172 = call "VIH UI - String Shortcut Menu Handler.vi"("Project Tree"=w269, "mode"=enum16{"basic", "format 1", "format 2"}."format 1", "menu"=w270, "Str Refnum"=w271, "Type"=w272) -> ()  [unwired: 7 in]
              n173 = event-data() -> ()  [unwired: 2 in, 1 out]
            }
            event "CtrlRule_Description": Shortcut Menu Selection (User) {
              n174 = event-data() -> ("Type"=w277:T23, "CtlRef"=w276:refnum<vi>, "ItemTag"=w274:string)  [unwired: 1 in, 1 out]
              n175 = call "VIH UI - String Shortcut Menu Handler.vi"("Project Tree"=w275, "Menu tag"=w274, "Str Refnum"=w276, "Type"=w277) -> ()  [unwired: 8 in]
            }
            event "Comments", "CtrlRule_CtrlID", "CtrlRule_CustomName": Shortcut Menu Activation? {
              n176 = event-data() -> ("Type"=w281:T23, "CtlRef"=w280:refnum<vi>, "MenuRef"=w279:refnum<k9>)  [unwired: 1 in, 1 out]
              n177 = call "VIH UI - String Shortcut Menu Handler.vi"("Project Tree"=w278, "mode"=enum16{"basic", "format 1", "format 2"}."basic", "menu"=w279, "Str Refnum"=w280, "Type"=w281) -> ()  [unwired: 7 in]
              n178 = event-data() -> ()  [unwired: 2 in, 1 out]
            }
            event "Comments", "CtrlRule_CtrlID", "CtrlRule_CustomName": Shortcut Menu Selection (User) {
              n179 = event-data() -> ("Type"=w286:T23, "CtlRef"=w285:refnum<vi>, "ItemTag"=w283:string)  [unwired: 1 in, 1 out]
              n180 = call "VIH UI - String Shortcut Menu Handler.vi"("Project Tree"=w284, "Menu tag"=w283, "Str Refnum"=w285, "Type"=w286) -> ()  [unwired: 8 in]
            }
          }
        }
      }
      frame "STARTUP" {
        w298 = i32[] [] ("CSS List")
        w299 = u32 16777216
        w305 = T24 {"Horizontal"=0, "Vertical"=0} ("Origin")
        w301 = T25 {"Left"=2, "Top"=0} ("Position")
        w297 = 1 ("CategoryList")
        n181 = control-ref of="JS List"() -> (w294:refnum<vi>)
        n182 = control-ref of="Category List"() -> (w288:refnum<vi>)
        n183 = control-ref of="CSS List"() -> (w295:refnum<vi>)
        n184 = property on="Pane-Top" class="Pane"("Origin"=w305) -> ()  [unwired: 2 in, 2 out]
        n185 = local write "CSS List"(w298) -> ()
        n186 = local write "Category List"(w297) -> ()
        n187 = property on="Pane-Left" class="Pane"("Origin"=w305) -> ()  [unwired: 2 in, 2 out]
        n188 = property on="Pane-Right" class="Pane"("Origin"=w305) -> ("Decos[]"=w304:refnum<vi>[])  [unwired: 2 in, 2 out]
        n189 = local write "JS List"(w298) -> ()
        n190 = Build Array(w295, w294) -> (w296:refnum<vi>[])
        n191 = local write "Tab Control"(w297) -> ()
        n192 = disable-structure shown="Disabled" {
          disable-tunnel: w296 -> [w312 _ _]
          disable-tunnel: w288 -> [_ w321 _]
          frame Disabled {
            n193 = call "VIH Utility - DEV - Get DevTime Utility VIs Folder.vi"("Utility VI Name"="Utility - Set File List Icons.vi") -> ("error out"=w317:errorcluster, "Utility VIs Path"=w316:path)  [unwired: 8 in, 1 out]
            n194 = Open VI Reference(type specifier VI Refnum (for type only)=refnum<vi> refnum, vi path=w316, error in (no error)=w317) -> (vi reference=w319:refnum<vi>, error out=w320:errorcluster)  [unwired: 3 in]
            n195 = call-by-ref "?"(reference=w319, error in=w320, "MCListbox Refnums"=w312) -> (reference out=w314:refnum<vi>, error out=w315:errorcluster, 0:"error out"=w311:errorcluster)  [unwired: 10 in]
            n196 = Close Reference(reference=w314, error in (no error)=w315) -> (error out=w310:errorcluster)
            n197 = Select(t=w310, s=w310, f=w311) -> (s? t:f=w313:errorcluster)
            n198 = call <vilib>:"Simple Error Handler.vi"("error in (no error)"=w313) -> ()  [unwired: 4 in, 5 out]
          }
          frame Disabled {
            n199 = call "VIH Utility - DEV - Get DevTime Utility VIs Folder.vi"("Utility VI Name"="Utility - Set Category List Text & Icons.vi") -> ("error out"=w329:errorcluster, "Utility VIs Path"=w328:path)  [unwired: 8 in, 1 out]
            n200 = Open VI Reference(type specifier VI Refnum (for type only)=refnum<vi> refnum, vi path=w328, error in (no error)=w329) -> (vi reference=w331:refnum<vi>, error out=w332:errorcluster)  [unwired: 3 in]
            n201 = call-by-ref "?"(reference=w331, error in=w332, "LstBox Refnum"=w321) -> (reference out=w326:refnum<vi>, error out=w327:errorcluster, 0:"error out"=w324:errorcluster)  [unwired: 10 in]
            n202 = Close Reference(reference=w326, error in (no error)=w327) -> (error out=w323:errorcluster)
            n203 = Select(t=w323, s=w323, f=w324) -> (s? t:f=w325:errorcluster)
            n204 = call <vilib>:"Simple Error Handler.vi"("error in (no error)"=w325) -> ()  [unwired: 4 in, 5 out]
          }
          frame Enabled {
          }
        }
        n205 = local write "CtrlRule List"(w298) -> ()
        n206 = Index Array(array=w304) -> (element=w306:refnum<vi>)  [unwired: 1 in]
        n207 = property class="Decor"(reference=w306, "Position"=w301) -> (error out=w302:errorcluster)  [unwired: 1 in, 1 out]
        n208 = property on="Tab Control" class="TabCtl (strict)"(error in=w302, "Position"=w301, "BG Color"=w299, "FG Color"=w299, "Tabs Visible?"=FALSE, "SkipTabbing"=TRUE ("Skip When Tabbing")) -> (error out=w303:errorcluster)  [unwired: 1 in, 1 out]
        n209 = property class="VI"() -> ("FP.State"=w291:T10)  [unwired: 2 in, 2 out]
        n210 = Close Reference(reference=w304, error in (no error)=w303) -> ()  [unwired: 1 out]
        n211 = call "VIH Debug Flag Container.vi"() -> ("Debug Mode"=w293:bool)  [unwired: 11 in]
        n212 = Equal?(x=w291, y=T10."Standard" ("Front Panel Window:State")) -> (x = y?=w289:bool)
        n213 = Or(x=w289, y=w293) -> (x .or. y?=w292:bool)
        n214 = property on="%STOP" class="Bool"("Visible"=w292) -> ()  [unwired: 2 in, 2 out]
        n215 = property on="%UPDATE" class="Bool"("Visible"=w292) -> ()  [unwired: 2 in, 2 out]
      }
      frame "INIT" {
        n216 = control-ref of="MenuDscrMode"() -> (w344:refnum<vi>)
        n217 = control-ref of="VIDscrMode"() -> (w343:refnum<vi>)
        n218 = control-ref of="VIDetailsMode"() -> (w342:refnum<vi>)
        n219 = control-ref of="PVIIDscrMode"() -> (w341:refnum<vi>)
        n220 = control-ref of="Ctl_DscrMode"() -> (w340:refnum<vi>)
        n221 = control-ref of="MenuItemIcons"() -> (w338:refnum<vi>)
        n222 = control-ref of="Ctl_ClustMembers"() -> (w337:refnum<vi>)
        n223 = control-ref of="Ctl_EnumValues"() -> (w336:refnum<vi>)
        n224 = Build Array(w338, w337, w336) -> (w335:refnum<vi>[])
        n225 = Build Array(w344, w343, w342, w341, w340) -> (w345:refnum<vi>[])
        n226 = Build Array(VIH_HelpGen_Typedef_-_Enum_-_Description_Mode."Default" ("element"), VIH_HelpGen_Typedef_-_Enum_-_Description_Mode."Custom" ("MenuDscrMode")) -> (w346:T3[])
        n227 = Build Array(VIH_HelpGen_Typedef_-_Enum_-_Default,Enable,Disable."Default" ("MenuItemIcons")) -> (w334:T2[])
        n228 = for {
          tunnel: w345 -> [w353] mode=indexing
          tunnel: w346 -> [w352]
          n229 = property class="Enum (strict)"(reference=w353, "Disabled Items []"=w352) -> ()  [unwired: 1 in, 2 out]
        }
        n230 = for {
          tunnel: w335 -> [w351] mode=indexing
          tunnel: w334 -> [w350]
          n231 = property class="Enum (strict)"(reference=w351, "Disabled Items []"=w350) -> ()  [unwired: 1 in, 2 out]
        }
      }
      frame "EXIT" {
        w357 = i32[] [] ("Item Symbols")
        w358 = string[][] [] ("Item Names")
        w359 = T26 {"Row"=0, "Column"=0} ("Top Left Visible Cell")
        n232 = control-ref of="Tab Control"() -> (w354:refnum<vi>)
        n233 = property class="TabCtl (strict)"(reference=w354, "DisabledEnum"=T11."Enabled" ("Disabled")) -> ("Pages"=w355:refnum<vi>[])  [unwired: 1 in, 2 out]
        n234 = property on="CtrlRule List" class="MCListbox (strict)"("TopLeft"=w359, "Value"=w357, "ItemNames"=w358, "ItemSyms"=w357) -> ()  [unwired: 2 in, 2 out]
        n235 = for {
          tunnel: w355 -> [w365] mode=indexing
          n236 = property class="Page"(reference=w365) -> (reference out=w363:refnum<vi>, "Controls on Page[]"=w364:refnum<vi>[])  [unwired: 1 in, 1 out]
          n237 = for {
            tunnel: w364 -> [w369] mode=indexing
            shift-right: [w366] -> w362
            shift-left: w363 -> [w366]
            n238 = property class="Ctl"(reference=w369, "DisabledEnum"=T11."Enabled" ("Disabled")) -> (reference out=w367:refnum<vi>)  [unwired: 1 in, 1 out]
            n239 = Close Reference(reference=w367) -> ()  [unwired: 1 in, 1 out]
          }
          n240 = Close Reference(reference=w362) -> ()  [unwired: 1 in, 1 out]
        }
        n241 = property on="CSS List" class="MCListbox (strict)"("TopLeft"=w359, "Value"=w357, "ItemNames"=w358, "ItemSyms"=w357) -> ()  [unwired: 2 in, 2 out]
        n242 = property on="JS List" class="MCListbox (strict)"("TopLeft"=w359, "Value"=w357, "ItemNames"=w358, "ItemSyms"=w357) -> ()  [unwired: 2 in, 2 out]
      }
      frame "HALT" {
        w370 = TRUE ("Visible")
        w371 = u32 16777238
        n243 = Unregister For Events(event registration refnum=w378) -> (error out=w376:errorcluster)  [unwired: 1 in]
        n244 = Destroy User Event(user event=w377, error in=w376) -> (error out=w374:errorcluster)
        n245 = Release Queue(queue=w375, error in (no error)=w374) -> ()  [unwired: 1 in, 3 out]
        n246 = property on="%STOP" class="Bool"("Visible"=w370) -> ()  [unwired: 2 in, 2 out]
        n247 = property on="Tab Control" class="TabCtl (strict)"("BG Color"=w371, "FG Color"=w371, "Tabs Visible?"=TRUE) -> ()  [unwired: 2 in, 2 out]
        n248 = property on="%UPDATE" class="Bool"("Visible"=w370) -> ()  [unwired: 2 in, 2 out]
      }
      frame "------------------------------ 1" {
      }
      frame "UPDATE" {
        n249 = Unbundle(w401) -> ("Array out"=w395:string[])  [unwired: 1 out]
        n250 = control-ref of="ProductInfoText"() -> (w393:refnum<vi>)
        n251 = control-ref of="Comments"() -> (w392:refnum<vi>)
        n252 = control-ref of="PI_Product"() -> (w390:refnum<vi>)
        n253 = control-ref of="PI_Version"() -> (w389:refnum<vi>)
        n254 = control-ref of="PI_Author"() -> (w388:refnum<vi>)
        n255 = control-ref of="PI_Company"() -> (w387:refnum<vi>)
        n256 = control-ref of="PI_Copyright"() -> (w386:refnum<vi>)
        n257 = control-ref of="PI_Website"() -> (w385:refnum<vi>)
        n258 = control-ref of="PI_Email"() -> (w384:refnum<vi>)
        n259 = control-ref of="PI_AddInfo"() -> (w383:refnum<vi>)
        n260 = case shown="\"REFRESH\"" w394 {
          selector: w394 -> [w410 _]
          tunnel: w395 -> [_ w412]
          tunnel: [w409 w412] -> w396
          frame Default {
            n261 = call "VIH Utility - STR - String to 1D Str Array.vi"("delimiter ('\\n')"="|" ("delimiter ('\\n')"), "String in"=w410) -> ("Array out"=w409:string[])  [unwired: 5 in]
          }
          frame "REFRESH" {
          }
        }
        n262 = Build Array(w393, w392, w390, w389, w388, w387, w386, w385, w384, w383) -> (w391:refnum<vi>[])
        n263 = Array Size(array=w396) -> (size(s)=w398:i32)
        n264 = for {
          tunnel: w391 -> [w407] mode=indexing
          n265 = property on="Property Node" class="Str"(reference=w407, "Text.Selection"=T12 {"Selection Start"=0, "Selection End"=0}) -> ()  [unwired: 1 in, 2 out]
        }
        n266 = Greater?(x=w398, y=1) -> (0:w400:bool)
        n267 = call "VIH Utility - UI - Boolean to Control Disable Status.vi"("Status in"=w400) -> ("Control Disable if True"=w397:u8)  [unwired: 3 in, 1 out]
        n268 = property on="Tab Control" class="TabCtl (strict)"("DisabledEnum"=w397) -> ()  [unwired: 2 in, 2 out]
        n269 = call "VIH Project - Container - Master Rule.vi"() -> ("Rule out"=w403:T15)  [unwired: 11 in]
        n270 = Bundle("Array out"=w396, "Rule out"=w403) -> (w402:cluster{"Array out":string[], "Rule out":T15})  [unwired: 1 in]
        n271 = Concatenate Strings("Update Category;\n\nSet Busy = ON;\n\nUpdate: UI;\nUpdate: Product Info;\nUpdate: General;\nUpdate: Target Paths;\nUpdate: Templates;\nUpdate: CSS List;\nUpdate: JS List;\nUpdate: Item Rules;\nUpdate: Control Rules;\n\nCSS List: Update Controls;\nJS List: Update Controls;\nCtrlRule: Update Controls = INIT;\n\nSet Busy = OFF;" ("string"), w406) -> (w405:string)
      }
      frame "Globals" {
        n272 = case shown="\"SET\"" w414 {
          tunnel: [w419 w422 w424] -> w417
          tunnel: w416 -> [w419 w421 w425]
          tunnel: w413 -> [w418 _ _]
          frame Default {
            n273 = One Button Dialog(message=w418) -> ()  [unwired: 1 in, 1 out]
          }
          frame "GET" {
            n274 = Unbundle(w421) -> ("Array out"=w420:string[])  [unwired: 1 out]
            n275 = call "VIH Project - Container - Master Rule.vi"() -> ("Rule out"=w423:T15)  [unwired: 11 in]
            n276 = Bundle("Array out"=w420, "Rule out"=w423) -> (w422:cluster{"Array out":string[], "Rule out":T15})  [unwired: 1 in]
          }
          frame "SET" {
            n277 = in-place {
              n278 = in-place-cluster #1(w425) -> ("Rule out"=w427:T15)
              n279 = call "VIH Project - Container - Master Rule.vi"("cmd (get)"=enum16{"get", "set"}."set", "Rule in"=w427) -> ("Rule out"=w426:T15)  [unwired: 9 in]
              n280 = in-place-cluster #1("Rule out"=w426) -> (w424:cluster{"Array out":string[], "Rule out":T15})
            }
          }
        }
      }
      frame "Update Category" {
        (unwired) "Project"
        n281 = property on="Category List" class="LstBox (strict)"() -> ("Item Names"=w436:string[])  [unwired: 2 in, 2 out]
        n282 = Index Array(array=w436, index=w435) -> (element=w433:string)
        n283 = To Unsigned Long Integer(number=w435) -> (unsigned 32bit integer=w431:u32)
        n284 = Concatenate Strings("Master Rule", " : " ("string"), w433) -> (→"CategoryTitle":string)
        n285 = property on="Tab Control" class="TabCtl (strict)"("Value"=w431) -> ()  [unwired: 2 in, 2 out]
      }
      frame "Set Busy" {
        n286 = case shown="\"ON\"" w438 {
          frame "OFF", Default {
            n287 = call <vilib>:"Unset Busy.vi"() -> ()  [unwired: 11 in, 1 out]
          }
          frame "ON" {
            n288 = call <vilib>:"Set Busy.vi"() -> ()  [unwired: 10 in, 2 out]
          }
        }
      }
      frame "Key Focus" {
        n289 = case shown="\"CtrlRule List\"" w442 {
          selector: w442 -> [w451 _ _ _ _ _]
          tunnel: [w451 _ _ _ _ _] -> w441
          frame Default {
          }
          frame "CtrlRule Control Name" {
            n290 = property on="CtrlRule_CtrlID" class="Str"("Key Focus"=TRUE, "Text.Selection End"=u32 9999 ("Text.Selection:End"), "Text.Selection Start"=u32 0 ("Text.Selection:Start")) -> ()  [unwired: 2 in, 2 out]
          }
          frame "CtrlRule List" {
            n291 = property on="CtrlRule List" class="MCListbox (strict)"("Key Focus"=TRUE) -> ()  [unwired: 2 in, 2 out]
          }
          frame "CSS List" {
            n292 = property on="CSS List" class="MCListbox (strict)"("Key Focus"=TRUE) -> ()  [unwired: 2 in, 2 out]
          }
          frame "JS List" {
            n293 = property on="JS List" class="MCListbox (strict)"("Key Focus"=TRUE) -> ()  [unwired: 2 in, 2 out]
          }
          frame "Category List" {
            n294 = property on="Category List" class="LstBox (strict)"("Key Focus"=TRUE) -> ()  [unwired: 2 in, 2 out]
          }
        }
        n295 = stacked-sequence {
          tunnel: w441 -> [_]
          frame #0 {
            n296 = control-ref of="CtrlRule List"() -> (w447:refnum<vi>)
            n297 = control-ref of="CSS List"() -> (w449:refnum<vi>)
            n298 = control-ref of="JS List"() -> (w448:refnum<vi>)
            n299 = control-ref of="Category List"() -> (w445:refnum<vi>)
            n300 = Build Array(w449, w448, w447) -> (w446:refnum<vi>[])
            n301 = for {
              tunnel: w446 -> [w450] mode=indexing
              n302 = call "VIH Utility - UI - Key Focus & Selection Color (MC Listbox).vi"("MCListbox Refnum"=w450) -> ()  [unwired: 8 in, 3 out]
            }
            n303 = call "VIH Utility - UI - Key Focus & Selection Color (Listbox).vi"("LstBox Refnum"=w445) -> ()  [unwired: 8 in, 3 out]
          }
        }
      }
      frame "------------------------------ 2" {
      }
      frame "Update: UI" {
        n304 = Unbundle(w462) -> ("Array out"=w466:string[])  [unwired: 1 out]
        n305 = Index Array(array=w466) -> (element=w464:string)  [unwired: 1 in]
        n306 = property class="Tree (strict)"(reference=w463, "Active Item Tag"=w464, "ActiveColNum"=0 ("Active Cell:Active Column Number")) -> ("Cell String"=→"Group Name":string)  [unwired: 1 in, 2 out]
      }
      frame "Update: Product Info" {
        n307 = Unbundle(w483) -> ("Rule out"=w482:T15)  [unwired: 1 out]
        n308 = Unbundle By Name(w482) -> ("ProductInfoMode"=w481:T2, "ProductInfoText"=w480:string)
        n309 = control-ref of="PI_Product"() -> (w477:refnum<vi>)
        n310 = control-ref of="PI_Version"() -> (w476:refnum<vi>)
        n311 = control-ref of="PI_Author"() -> (w475:refnum<vi>)
        n312 = control-ref of="PI_Company"() -> (w474:refnum<vi>)
        n313 = control-ref of="PI_Copyright"() -> (w473:refnum<vi>)
        n314 = control-ref of="PI_Website"() -> (w472:refnum<vi>)
        n315 = control-ref of="PI_Email"() -> (w471:refnum<vi>)
        n316 = control-ref of="PI_AddInfo"() -> (w470:refnum<vi>)
        n317 = Not Equal?(x=w481, y=VIH_HelpGen_Typedef_-_Enum_-_Default,Enable,Disable."Enable") -> (x != y?=w485:bool)
        n318 = Build Array(w477, w476, w475, w474, w473, w472, w471, w470) -> (w469:refnum<vi>[])
        n319 = call "VIH Project - Container - Product Info.vi"() -> ("Product Info out"=w478:T27)  [unwired: 11 in]
        n320 = call "VIH Utility - UI - Boolean to Control Disable Status.vi"("Status in"=w485) -> ("Control Disable if True"=w479:u8)  [unwired: 3 in, 1 out]
        n321 = Cluster To Array(cluster=w478) -> (array=w468:string[])
        n322 = for {
          tunnel: w469 -> [w488] mode=indexing
          tunnel: w468 -> [w487] mode=indexing
          n323 = property class="Str"(reference=w488, "Value"=w487) -> ()  [unwired: 1 in, 2 out]
        }
        n324 = property on="ProductInfoMode" class="Enum (strict)"("Value"=w481) -> ()  [unwired: 2 in, 2 out]
        n325 = property on="ProductInfoText" class="Str"("DisabledEnum"=w479, "Value"=w480) -> ()  [unwired: 2 in, 2 out]
      }
      frame "Update: General" {
        n326 = Unbundle(w491) -> ("Rule out"=w490:T15)  [unwired: 1 out]
        n327 = Unbundle By Name(w490) -> ("%Comments"=w489:string)  [unwired: 1 out]
        n328 = local write "Comments"(w489) -> ()
      }
      frame "Update: Target Paths" {
        w494 = FALSE ("Allow Empty Path (T)")
        n329 = Unbundle(w513) -> ("Rule out"=w512:T15)  [unwired: 1 out]
        n330 = Unbundle By Name(w512) -> ("Build Root Dir"=w493:path, "Target Paths"=w511:T17)
        n331 = Unbundle By Name(w511) -> ("HTML Dir"=w504:path, "Image Dir"=w506:path, "CSS Dir"=w508:path, "JS Dir"=w510:path)
        n332 = disable-structure shown="Disabled" {
          disable-tunnel: w510 -> [w526 w531]
          disable-tunnel: [w525 _] -> w509
          disable-tunnel: [w524 w531] -> w495
          disable-tunnel: w508 -> [w523 w532]
          disable-tunnel: [w522 w532] -> w496
          disable-tunnel: [w521 _] -> w507
          disable-tunnel: w506 -> [w520 w533]
          disable-tunnel: [w519 w533] -> w497
          disable-tunnel: [w518 _] -> w505
          disable-tunnel: w504 -> [w517 w534]
          disable-tunnel: [w516 w534] -> w498
          disable-tunnel: [w515 _] -> w503
          frame Disabled {
            n333 = call "VIH UI - Test Path.vi"("Folder (F)"=TRUE, "Path"=w517) -> ("Color"=w515:u32, "dup Path"=w516:path)  [unwired: 6 in, 2 out]
            n334 = call "VIH UI - Test Path.vi"("Folder (F)"=TRUE, "Path"=w523) -> ("Color"=w521:u32, "dup Path"=w522:path)  [unwired: 6 in, 2 out]
            n335 = call "VIH UI - Test Path.vi"("Folder (F)"=TRUE, "Path"=w520) -> ("Color"=w518:u32, "dup Path"=w519:path)  [unwired: 6 in, 2 out]
            n336 = call "VIH UI - Test Path.vi"("Folder (F)"=TRUE, "Path"=w526) -> ("Color"=w525:u32, "dup Path"=w524:path)  [unwired: 6 in, 2 out]
          }
          frame Enabled {
          }
        }
        n337 = call "VIH HelpGen - FILE - Build Absolute Path.vi"("Root Path"=w493, "Allow Empty Path (T)"=w494, "Path in"=w498) -> ("Path out"=w499:path)  [unwired: 8 in]
        n338 = call "VIH HelpGen - FILE - Build Absolute Path.vi"("Root Path"=w493, "Allow Empty Path (T)"=w494, "Path in"=w497) -> ("Path out"=w500:path)  [unwired: 8 in]
        n339 = call "VIH HelpGen - FILE - Build Absolute Path.vi"("Root Path"=w493, "Allow Empty Path (T)"=w494, "Path in"=w496) -> ("Path out"=w501:path)  [unwired: 8 in]
        n340 = call "VIH HelpGen - FILE - Build Absolute Path.vi"("Root Path"=w493, "Allow Empty Path (T)"=w494, "Path in"=w495) -> ("Path out"=w502:path)  [unwired: 8 in]
        n341 = property on="Dst_HTML Dir" class="Path"("Value"=w498, "Text.TextColor"=w503, "StartPath"=w499) -> ()  [unwired: 2 in, 2 out]
        n342 = property on="Dst_Image Dir" class="Path"("Value"=w497, "Text.TextColor"=w505, "StartPath"=w500) -> ()  [unwired: 2 in, 2 out]
        n343 = property on="Dst_CSS Dir" class="Path"("Value"=w496, "Text.TextColor"=w507, "StartPath"=w501) -> ()  [unwired: 2 in, 2 out]
        n344 = property on="Dst_JS Dir" class="Path"("Value"=w495, "Text.TextColor"=w509, "StartPath"=w502) -> ()  [unwired: 2 in, 2 out]
        n345 = property on="Build Root Dir" class="Path"("Value"=w493) -> ()  [unwired: 2 in, 2 out]
      }
      frame "Update: Templates" {
        n346 = Unbundle(w546) -> ("Rule out"=w545:T15)  [unwired: 1 out]
        n347 = Unbundle By Name(w545) -> ("Source Paths"=w544:T16)
        n348 = Unbundle By Name(w544) -> ("VI Template"=w542:path, "Menu Template"=w543:path, "PolyVI Template"=w535:path)
        n349 = call "VIH UI - Test Path.vi"("Path"=w542) -> ("Color"=w540:u32, "dup Path"=w541:path)  [unwired: 7 in, 2 out]
        n350 = call "VIH UI - Test Path.vi"("Path"=w543) -> ("Color"=w538:u32, "dup Path"=w539:path)  [unwired: 7 in, 2 out]
        n351 = call "VIH UI - Test Path.vi"("Path"=w535) -> ("Color"=w536:u32, "dup Path"=w537:path)  [unwired: 7 in, 2 out]
        n352 = property on="Src_PolyVI Template" class="Path"("Value"=w537, "Text.TextColor"=w536) -> ()  [unwired: 2 in, 2 out]
        n353 = property on="Src_VI Template" class="Path"("Value"=w541, "Text.TextColor"=w540) -> ()  [unwired: 2 in, 2 out]
        n354 = property on="Src_Menu Template" class="Path"("Value"=w539, "Text.TextColor"=w538) -> ()  [unwired: 2 in, 2 out]
      }
      frame "Update: CSS List" {
        n355 = Unbundle(w562) -> ("Rule out"=w561:T15)  [unwired: 1 out]
        n356 = Unbundle By Name(w561) -> ("Source Paths"=w560:T16)
        n357 = Unbundle By Name(w560) -> ("CSS Files"=w559:path[])
        n358 = for {
          tunnel: w559 -> [w565] mode=indexing
          tunnel: [w564] -> w550 mode=indexing
          tunnel: [w566] -> w558 mode=indexing
          n359 = Path To String(path=w565) -> (string=w567:string)
          n360 = call "VIH UI - Test Path.vi"("Path"=w565) -> ("Symbol"=w564:i32)  [unwired: 7 in, 3 out]
          n361 = Build Array(w567) -> (w566:string[])
        }
        n362 = Not Equal?(x=w550, y=0) -> (x != y?=w549:bool[])
        n363 = Or Array Elements(Boolean array=w549) -> (logical OR=w548:bool)
        n364 = call "VIH Utility - UI - Drag and Drop Supporter (w Symbol Indices).vi"("Cmd"=enum16{"make symbols", "test D'n'D"}."make symbols", "Item Symbols"=w550) -> ("Item Symbols out"=w556:i32[])  [unwired: 7 in, 2 out]
        n365 = control-ref of="CSS List"() -> (w555:refnum<vi>)
        n366 = Index Array(array=w553) -> (element=w552:i32)  [unwired: 1 in]
        n367 = property on="CSS List" class="MCListbox (strict)"("ItemNames"=w558, "ItemSyms"=w556, "Symbols Vis"=w548) -> (error out=w554:errorcluster)  [unwired: 2 in, 1 out]
        n368 = call "VIH Utility - UI - Make Row Visible (MC Listbox).vi"("error in"=w554, "Row"=w552, "MC Listbox Refnum"=w555) -> ()  [unwired: 7 in, 2 out]
      }
      frame "Update: JS List" {
        n369 = Unbundle(w582) -> ("Rule out"=w581:T15)  [unwired: 1 out]
        n370 = Unbundle By Name(w581) -> ("Source Paths"=w580:T16)
        n371 = Unbundle By Name(w580) -> ("JS Files"=w579:path[])
        n372 = for {
          tunnel: w579 -> [w585] mode=indexing
          tunnel: [w584] -> w569 mode=indexing
          tunnel: [w586] -> w578 mode=indexing
          n373 = Path To String(path=w585) -> (string=w587:string)
          n374 = call "VIH UI - Test Path.vi"("Path"=w585) -> ("Symbol"=w584:i32)  [unwired: 7 in, 3 out]
          n375 = Build Array(w587) -> (w586:string[])
        }
        n376 = Not Equal?(x=w569, y=0) -> (x != y?=w570:bool[])
        n377 = Or Array Elements(Boolean array=w570) -> (logical OR=w568:bool)
        n378 = control-ref of="JS List"() -> (w575:refnum<vi>)
        n379 = Index Array(array=w573) -> (element=w572:i32)  [unwired: 1 in]
        n380 = call "VIH Utility - UI - Drag and Drop Supporter (w Symbol Indices).vi"("Cmd"=enum16{"make symbols", "test D'n'D"}."make symbols", "Item Symbols"=w569) -> ("Item Symbols out"=w576:i32[])  [unwired: 7 in, 2 out]
        n381 = property on="JS List" class="MCListbox (strict)"("ItemNames"=w578, "ItemSyms"=w576, "Symbols Vis"=w568) -> (error out=w574:errorcluster)  [unwired: 2 in, 1 out]
        n382 = call "VIH Utility - UI - Make Row Visible (MC Listbox).vi"("error in"=w574, "Row"=w572, "MC Listbox Refnum"=w575) -> ()  [unwired: 7 in, 2 out]
      }
      frame "Update: Item Rules" {
        n383 = Unbundle(w597) -> ("Rule out"=w590:T15)  [unwired: 1 out]
        n384 = Unbundle By Name(w590) -> ("Ctl_DscrMode"=w593:T3, "Ctl_ClustMembers"=w592:T2, "Ctl_EnumValues"=w591:T2)
        n385 = Unbundle By Name(w590) -> ("VIDscrMode"=w596:T3, "MenuDscrMode"=w595:T3, "MenuItemIcons"=w594:T2, "PVIIDscrMode"=w589:T3, "VIDetailsMode"=w588:T3)
        n386 = local write "VIDscrMode"(w596) -> ()
        n387 = local write "MenuDscrMode"(w595) -> ()
        n388 = local write "MenuItemIcons"(w594) -> ()
        n389 = local write "PVIIDscrMode"(w589) -> ()
        n390 = local write "VIDetailsMode"(w588) -> ()
        n391 = local write "Ctl_DscrMode"(w593) -> ()
        n392 = local write "Ctl_ClustMembers"(w592) -> ()
        n393 = local write "Ctl_EnumValues"(w591) -> ()
      }
      frame "Update: Control Rules" {
        n394 = Unbundle(w609) -> ("Rule out"=w608:T15)  [unwired: 1 out]
        n395 = Unbundle By Name(w608) -> ("Control Rules"=w607:T18[])
        n396 = for {
          tunnel: w607 -> [w622] mode=indexing
          tunnel: [w620] -> w606 mode=indexing
          tunnel: [w616] -> w605 mode=indexing
          n397 = Unbundle By Name(w622) -> ("CtrlID"=w621:string, "CustomRule"=w619:bool, "EnumValDscr"=w615:T19[])
          n398 = Empty Array?(array=w615) -> (empty?=w614:bool)
          n399 = Select(t="", s=w614, f="VList") -> (s? t:f=w611:string)
          n400 = Select(t=38, s=w619, f=37) -> (s? t:f=w616:i32)
          n401 = Build Array(w621, w611) -> (w620:string[])
        }
        n402 = control-ref of="CtrlRule List"() -> (w601:refnum<vi>)
        n403 = Index Array(array=w600) -> (element=w599:i32)  [unwired: 1 in]
        n404 = call "VIH Utility - UI - Drag and Drop Supporter (w Symbol Indices).vi"("Cmd"=enum16{"make symbols", "test D'n'D"}."make symbols", "Item Symbols"=w605) -> ("Item Symbols out"=w604:i32[])  [unwired: 7 in, 2 out]
        n405 = property on="CtrlRule List" class="MCListbox (strict)"("ItemNames"=w606, "ItemSyms"=w604) -> (error out=w602:errorcluster)  [unwired: 2 in, 1 out]
        n406 = call "VIH Utility - UI - Make Row Visible (MC Listbox).vi"("error in"=w602, "Row"=w599, "MC Listbox Refnum"=w601) -> ()  [unwired: 7 in, 2 out]
      }
      frame "------------------------------ 3" {
      }
      frame "Apply: Product Info" {
        n407 = Unbundle(w642) -> ("Array out"=w641:string[], "Rule out"=w639:T15)
        n408 = in-place {
          n409 = in-place-cluster #2(w639) -> ()  [unwired: 2 out]
          n410 = in-place-cluster #2("ProductInfoMode"="ProductInfoMode", "ProductInfoText"="ProductInfoText") -> (w638:T15)
        }
        n411 = call "VIH Project - Container - Product Info.vi"() -> ("Product Info out"=w635:T27)  [unwired: 11 in]
        n412 = Bundle By Name(cluster=w635, "ProductName"="PI_Product", "Version"="PI_Version", "Author"="PI_Author", "Company"="PI_Company", "Copyright"="PI_Copyright", "Website"="PI_Website", "Email"="PI_Email", "AddInfo"="PI_AddInfo") -> (w626:T27)
        n413 = call "VIH Project - Container - Product Info.vi"("cmd (get)"=enum16{"get", "set"}."set", "Product Info in"=w626) -> ()  [unwired: 9 in, 1 out]
        n414 = Concatenate Strings("Globals = Set;\nUpdate: Product Info;" ("string"), w643) -> (w637:string)
        n415 = Bundle("Array out"=w641, "Rule out"=w638) -> (w640:cluster{"Array out":string[], "Rule out":T15})  [unwired: 1 in]
      }
      frame "Apply: General" {
        n416 = Unbundle(w652) -> ("Array out"=w651:string[], "Rule out"=w649:T15)
        n417 = in-place {
          n418 = in-place-cluster #3(w649) -> ()  [unwired: 2 out]
          n419 = in-place-cluster #3("Source Root Dir"=path "", "%Comments"="Comments") -> (w648:T15)
        }
        n420 = Concatenate Strings("Globals = Set;\nUpdate: General;" ("string"), w653) -> (w647:string)
        n421 = Bundle("Array out"=w651, "Rule out"=w648) -> (w650:cluster{"Array out":string[], "Rule out":T15})  [unwired: 1 in]
      }
      frame "Apply: Target Paths" {
        n422 = Unbundle(w663) -> ("Array out"=w662:string[], "Rule out"=w660:T15)
        n423 = in-place {
          n424 = in-place-cluster #4(w660) -> ()  [unwired: 5 out]
          n425 = in-place-cluster #4("Build Root Dir"="Build Root Dir", "Target Paths.HTML Dir"="Dst_HTML Dir", "Target Paths.Image Dir"="Dst_Image Dir", "Target Paths.CSS Dir"="Dst_CSS Dir", "Target Paths.JS Dir"="Dst_JS Dir") -> (w659:T15)
        }
        n426 = Concatenate Strings("Globals = Set;\nUpdate: Target Paths;" ("string"), w657) -> (w656:string)
        n427 = Bundle("Array out"=w662, "Rule out"=w659) -> (w661:cluster{"Array out":string[], "Rule out":T15})  [unwired: 1 in]
      }
      frame "Apply: Templates" {
        n428 = Unbundle(w676) -> ("Array out"=w675:string[], "Rule out"=w673:T15)
        n429 = in-place {
          n430 = in-place-cluster #5(w673) -> ()  [unwired: 3 out]
          n431 = call "VIH Project - Container - Project File Path.vi"() -> ("Project File Path"=w687:path)  [unwired: 9 in, 2 out]
          n432 = call "VIH Project - Get Default Template File Path.vi"("Template Type"=enum16{"menu", "VI", "PolyVI"}."VI", "Path"="Src_VI Template") -> ("Path out"=w684:path)  [unwired: 9 in]
          n433 = call "VIH Project - Get Default Template File Path.vi"("Template Type"=enum16{"menu", "VI", "PolyVI"}."menu", "Path"="Src_Menu Template") -> ("Path out"=w682:path)  [unwired: 9 in]
          n434 = call "VIH Project - Get Default Template File Path.vi"("Template Type"=enum16{"menu", "VI", "PolyVI"}."PolyVI", "Path"="Src_PolyVI Template") -> ("Path out"=w680:path)  [unwired: 9 in]
          n435 = Strip Path(path=w687) -> (stripped path=w686:path)  [unwired: 1 out]
          n436 = call "VIH HelpGen - FILE - Build Absolute Path.vi"("Root Path"=w686, "Allow Empty Path (T)"=FALSE, "Path in"=w684) -> ("Path out"=w690:path)  [unwired: 8 in]
          n437 = call "VIH HelpGen - FILE - Build Absolute Path.vi"("Root Path"=w686, "Allow Empty Path (T)"=FALSE, "Path in"=w682) -> ("Path out"=w688:path)  [unwired: 8 in]
          n438 = call "VIH HelpGen - FILE - Build Absolute Path.vi"("Root Path"=w686, "Allow Empty Path (T)"=FALSE, "Path in"=w680) -> ("Path out"=w689:path)  [unwired: 8 in]
          n439 = in-place-cluster #5("Source Paths.VI Template"=w690, "Source Paths.Menu Template"=w688, "Source Paths.PolyVI Template"=w689) -> (w672:T15)
        }
        n440 = Concatenate Strings("Globals = Set;\nUpdate: Templates;" ("string"), w670) -> (w669:string)
        n441 = Bundle("Array out"=w675, "Rule out"=w672) -> (w674:cluster{"Array out":string[], "Rule out":T15})  [unwired: 1 in]
      }
      frame "Apply: Item Rules" {
        n442 = Unbundle(w701) -> ("Array out"=w700:string[], "Rule out"=w698:T15)
        n443 = in-place {
          n444 = in-place-cluster #6(w698) -> ()  [unwired: 8 out]
          n445 = in-place-cluster #6("VIDscrMode"="VIDscrMode", "MenuDscrMode"="MenuDscrMode", "MenuItemIcons"="MenuItemIcons", "Ctl_DscrMode"="Ctl_DscrMode", "Ctl_ClustMembers"="Ctl_ClustMembers", "Ctl_EnumValues"="Ctl_EnumValues", "PVIIDscrMode"="PVIIDscrMode", "VIDetailsMode"="VIDetailsMode") -> (w697:T15)
        }
        n446 = Concatenate Strings("Globals = Set;\nUpdate: Item Rules;" ("string"), w695) -> (w694:string)
        n447 = Bundle("Array out"=w700, "Rule out"=w697) -> (w699:cluster{"Array out":string[], "Rule out":T15})  [unwired: 1 in]
      }
      frame "------------------------------ 4" {
      }
      frame "CtrlRule: Update Controls" {
        n448 = Unbundle(w728) -> ("Rule out"=w727:T15)  [unwired: 1 out]
        n449 = Array Size(array=w718) -> (size(s)=w716:i32)
        n450 = Index Array(array=w718) -> (element=w717:i32)  [unwired: 1 in]
        n451 = Unbundle By Name(w727) -> ("Control Rules"=w726:T18[])
        n452 = case shown="\"INIT\"" w712 {
          frame Default {
          }
          frame "INIT" {
            n453 = control-ref of="CtrlRule_CtrlID"() -> (w732:refnum<vi>)
            n454 = control-ref of="CtrlRule_CustomName"() -> (w731:refnum<vi>)
            n455 = control-ref of="CtrlRule_Description"() -> (w730:refnum<vi>)
            n456 = Build Array(w732, w731, w730) -> (w733:refnum<vi>[])
            n457 = for {
              tunnel: w733 -> [w734] mode=indexing
              n458 = property on="Property Node" class="Str"(reference=w734, "Text.Selection"=T12 {"Selection Start"=0, "Selection End"=0}) -> ()  [unwired: 1 in, 2 out]
            }
          }
        }
        n459 = case shown="1" w716 {
          tunnel: w717 -> [_ w749 _]
          tunnel: w726 -> [_ w748 _]
          tunnel: [_ w746 _] -> w725
          tunnel: [_ w745 _] -> w724
          tunnel: [_ w741 _] -> w723
          tunnel: [_ w744 _] -> w722
          tunnel: [_ w743 _] -> w721
          tunnel: [_ w742 _] -> w720
          tunnel: [w736 _ w750] -> w714
          tunnel: [w736 w739 w750] -> w719
          tunnel: [w736 _ _] -> w715
          tunnel: [_ w737 _] -> w713
          frame ..0 {
            w736 = u8 2
          }
          frame 1 {
            n460 = Index Array(array=w748, index=w749) -> (element=w747:T18)
            n461 = Unbundle By Name(w747) -> ("CtrlID"=w746:string, "CustomRule"=w745:bool, "DscrMode"=w741:T3, "Description"=w744:string, "ClusterMembers"=w743:T2, "EnumValues"=w742:T2, "CustomName"=w737:string)
            n462 = Equal?(x=VIH_HelpGen_Typedef_-_Enum_-_Description_Mode."Custom", y=w741) -> (x = y?=w738:bool)
            n463 = call "VIH Utility - UI - Boolean to Control Disable Status.vi"("Status in"=w738) -> ("Control Disable if False"=w739:u8)  [unwired: 3 in, 1 out]
          }
          frame 2.. {
            w750 = u8 2
          }
        }
        n464 = property on="%CtrlRule_Copy" class="Bool"("DisabledEnum"=w715) -> ()  [unwired: 2 in, 2 out]
        n465 = property on="CtrlRule_CtrlID" class="Str"("DisabledEnum"=w714, "Value"=w725) -> ()  [unwired: 2 in, 2 out]
        n466 = property on="CtrlRule_DscrMode" class="Enum (strict)"("DisabledEnum"=w714, "Value"=w723) -> ()  [unwired: 2 in, 2 out]
        n467 = property on="CtrlRule_ClusterMembers" class="Enum (strict)"("DisabledEnum"=w714, "Value"=w721) -> ()  [unwired: 2 in, 2 out]
        n468 = property on="CtrlRule_CustomName" class="Str"("DisabledEnum"=w714, "Value"=w713) -> ()  [unwired: 2 in, 2 out]
        n469 = property on="CtrlRule_CustomRule" class="Bool (strict)"("DisabledEnum"=w714, "Value"=w724) -> ()  [unwired: 2 in, 2 out]
        n470 = property on="CtrlRule_Description" class="Str"("DisabledEnum"=w719, "Value"=w722) -> ()  [unwired: 2 in, 2 out]
        n471 = property on="CtrlRule_EnumValues" class="Enum (strict)"("DisabledEnum"=w714, "Value"=w720) -> ()  [unwired: 2 in, 2 out]
        n472 = property on="%CtrlRule_Remove" class="Bool"("DisabledEnum"=w715) -> ()  [unwired: 2 in, 2 out]
        n473 = property on="%CtrlRule_Edit_Enum" class="Bool"("DisabledEnum"=w714) -> ()  [unwired: 2 in, 2 out]
      }
      frame "CtrlRule: Add" {
        n474 = Unbundle(w761) -> ("Rule out"=w763:T15)  [unwired: 1 out]
        n475 = Array Size(array=w752) -> (size(s)=w757:i32)
        n476 = Array Max & Min(array=w752) -> (max value=w755:i32)  [unwired: 3 out]
        n477 = Less Or Equal To 0?(x=w757) -> (x <= 0?=w756:bool)
        n478 = Select(t=-1, s=w756, f=w755) -> (s? t:f=w753:i32)
        n479 = Increment(x=w753) -> (x+1=w751:i32)
        n480 = in-place {
          in-place-border: w751 -> [w765]
          n481 = in-place-cluster #7(w763) -> ("Control Rules"=w773:T18[])
          n482 = Array Size(array=w773) -> (size(s)=w774:i32)
          n483 = Index Array(array=w773, index=-1) -> (element=w771:T18)
          n484 = In Range and Coerce(upper limit=w774, x=w765, lower limit=0) -> (coerced(x)=w772:i32)  [unwired: 1 out]
          n485 = Bundle By Name(cluster=w771, "CtrlID"="<Control Name>", "CustomRule"=TRUE) -> (w770:T18)
          n486 = Build Array(w772) -> (w766:i32[])
          n487 = local write "CtrlRule List"(w766) -> ()
          n488 = Insert Into Array(array=w773, index=w772, new element=w770) -> (w776:T18[])
          n489 = in-place-cluster #7("Control Rules"=w776) -> (w762:T15)
        }
        n490 = Concatenate Strings("Globals = Set;\n\nUpdate: Control Rules;\nCtrlRule: Update Controls = INIT;" ("string"), w764) -> (w759:string)
        n491 = Bundle(cluster=w761, "Rule out"=w762) -> (w760:cluster{"Array out":string[], "Rule out":T15})  [unwired: 1 in]
      }
      frame "CtrlRule: Import" {
        n492 = case shown="\"VI\", Default" w781 {
          tunnel: [w799 w803] -> w783
          tunnel: [TRUE w802] -> w780
          tunnel: w779 -> [w790 _]
          tunnel: [w789 -1] -> w778
          tunnel: w777 -> [_ w801]
          frame "CB", "Clipboard" {
            n493 = invoke class="App" method="Clipboard.Read"() -> ("Read Clipbrd"=w798:string)  [unwired: 3 in, 2 out]
            n494 = Array Size(array=w790) -> (size(s)=w795:i32)
            n495 = Array Max & Min(array=w790) -> (max value=w791:i32)  [unwired: 3 out]
            n496 = Less Or Equal To 0?(x=w795) -> (x <= 0?=w794:bool)
            n497 = Select(t=-1, s=w794, f=w791) -> (s? t:f=w792:i32)
            n498 = call "VIH XML - Control Rules to-from XML String.vi"("cmd (check)"=enum16{"check", "parse", "format"}."parse", "XML in"=w798) -> ("Control Rules out"=w799:T18[])  [unwired: 6 in, 3 out]
            n499 = Increment(x=w792) -> (x+1=w789:i32)
          }
          frame "VI", Default {
            n500 = call "VIH Dialog - Project File List.vi"("Ena Custom VI (F)"=TRUE, "File set (All)"=enum32{"ALL", "conpane", "invalid"}."conpane", "Project Tree"=w801) -> ("OK out"=w805:bool, "File Path"=w806:path)  [unwired: 6 in, 1 out]
            n501 = case shown="True" w805 {
              tunnel: w806 -> [_ w811]
              tunnel: [_ w810] -> w802
              tunnel: [_ w809] -> _
              tunnel: [_ w808] -> w803
              frame False {
              }
              frame True {
                n502 = call "VIH Dialog - VI Terminals.vi"("VI Path"=w811) -> ("OK out"=w810:bool, "Ctrl Rules"=w808:T18[], "Ctrl IDs out"=w809:string[])  [unwired: 7 in, 1 out]
              }
            }
          }
        }
        n503 = Empty Array?(array=w783) -> (empty?=w782:bool)
        n504 = case shown="False" w782 {
          tunnel: w787 -> [w816 w825]
          tunnel: [w815 w825] -> w784
          tunnel: ["Globals = Set;\n\nUpdate: Control Rules;\nCtrlRule: Update Controls = INIT;" ("string") _] -> w788
          tunnel: w783 -> [w813 _]
          tunnel: w780 -> [_ w824]
          tunnel: w778 -> [w812 _]
          frame False {
            n505 = Unbundle(w816) -> ("Rule out"=w818:T15)  [unwired: 1 out]
            n506 = in-place {
              in-place-border: w813 -> [w821]
              in-place-border: w812 -> [w819]
              n507 = in-place-cluster #8(w818) -> ("Control Rules"=w823:T18[])
              n508 = call "VIH UI - Append Control Rules.vi"("Position Index (-1)"=w819, "Ctrl Rules (new)"=w821, "Ctrl Rules (existing)"=w823) -> ("Indices"=w820:i32[], "Ctrl Rules out"=w822:T18[])  [unwired: 7 in]
              n509 = in-place-cluster #8("Control Rules"=w822) -> (w817:T15)
              n510 = property on="CtrlRule List" class="MCListbox (strict)"("Value"=w820) -> ()  [unwired: 2 in, 2 out]
            }
            n511 = Bundle(cluster=w816, "Rule out"=w817) -> (w815:cluster{"Array out":string[], "Rule out":T15})  [unwired: 1 in]
          }
          frame True {
            n512 = case shown="True" w824 {
              frame False {
              }
              frame True {
                n513 = call <vilib>:"Beep.vi"() -> ()  [unwired: 12 in]
              }
            }
          }
        }
        n514 = Concatenate Strings(w788, w786) -> (w785:string)
      }
      frame "CtrlRule: Export" {
        n515 = Unbundle(w829) -> ("Rule out"=w830:T15)  [unwired: 1 out]
        n516 = Unbundle By Name(w830) -> ("Control Rules"=w828:T18[])
        n517 = for {
          tunnel: w827 -> [w838] mode=indexing
          tunnel: w828 -> [w837]
          tunnel: [w836] -> w826 mode=indexing
          n518 = Index Array(array=w837, index=w838) -> (element=w836:T18)
        }
        n519 = call "VIH XML - Control Rules to-from XML String.vi"("cmd (check)"=enum16{"check", "parse", "format"}."format", "Control Rules in"=w826) -> ("error out"=w832:errorcluster, "XML out"=w833:string)  [unwired: 6 in, 2 out]
        n520 = invoke class="App" method="Clipboard.Write"(error in=w832, "Param 0"=w833) -> (error out=w834:errorcluster)  [unwired: 2 in, 3 out]
        n521 = call <vilib>:"Simple Error Handler.vi"("error in (no error)"=w834) -> ()  [unwired: 4 in, 5 out]
      }
      frame "CtrlRule: Remove" {
        n522 = Unbundle(w846) -> ("Rule out"=w839:T15)  [unwired: 1 out]
        n523 = in-place {
          in-place-border: w840 -> [w851]
          in-place-border: [w848] -> w841
          n524 = in-place-cluster #9(w839) -> ("Control Rules"=w850:T18[])
          n525 = Sort 1D Array(array=w851) -> (sorted array=w852:i32[])
          n526 = Reverse 1D Array(array=w852) -> (reversed array=w861:i32[])
          n527 = for {
            tunnel: w861 -> [w862] mode=indexing
            shift-right: [w864] -> w849
            shift-left: w850 -> [w863]
            n528 = Delete From Array(array=w863, index=w862) -> (array with subset deleted=w864:T18[])  [unwired: 1 in, 1 out]
          }
          n529 = Index Array(array=w852) -> (element=w860:i32)  [unwired: 1 in]
          n530 = Array Size(array=w849) -> (size(s)=w858:i32)
          n531 = Decrement(x=w858) -> (x-1=w853:i32)
          n532 = In Range and Coerce(upper limit=w853, x=w860, lower limit=0) -> (coerced(x)=w856:i32)  [unwired: 1 out]
          n533 = Less Than 0?(x=w853) -> (x < 0?=w857:bool)
          n534 = Build Array(w856) -> (w855:i32[])
          n535 = Select(t=i32[] [] ("CSS List"), s=w857, f=w855) -> (s? t:f=w848:i32[])
          n536 = in-place-cluster #9("Control Rules"=w849) -> (w842:T15)
        }
        n537 = Concatenate Strings("Globals = Set;\n\nUpdate: Control Rules;\nCtrlRule: Update Controls = INIT;" ("string"), w847) -> (w844:string)
        n538 = local write "CtrlRule List"(w841) -> ()
        n539 = Bundle(cluster=w846, "Rule out"=w842) -> (w845:cluster{"Array out":string[], "Rule out":T15})  [unwired: 1 in]
      }
      frame "CtrlRule: Dragged" {
        n540 = Unbundle(w868) -> ("Rule out"=w870:T15)  [unwired: 1 out]
        n541 = in-place {
          n542 = in-place-cluster #10(w870) -> ("Control Rules"=w873:T18[])
          n543 = property on="CtrlRule List" class="MCListbox (strict)"() -> ("ItemSyms"=w876:i32[])  [unwired: 2 in, 2 out]
          n544 = call "VIH Utility - UI - Drag and Drop Supporter (w Symbol Indices).vi"("Cmd"=enum16{"make symbols", "test D'n'D"}."test D'n'D", "Item Symbols"=w876) -> ("indices"=w874:i32[])  [unwired: 7 in, 2 out]
          n545 = for {
            tunnel: w874 -> [w879] mode=indexing
            tunnel: w873 -> [w878]
            tunnel: [w877] -> w872 mode=indexing
            n546 = Index Array(array=w878, index=w879) -> (element=w877:T18)
          }
          n547 = in-place-cluster #10("Control Rules"=w872) -> (w869:T15)
        }
        n548 = Concatenate Strings("Globals = Set;\n\nUpdate: Control Rules;\nCtrlRule: Update Controls = INIT;" ("string"), w871) -> (w866:string)
        n549 = Bundle(cluster=w868, "Rule out"=w869) -> (w867:cluster{"Array out":string[], "Rule out":T15})  [unwired: 1 in]
      }
      frame "CtrlRule: Apply" {
        n550 = Unbundle(w885) -> ("Rule out"=w887:T15)  [unwired: 1 out]
        n551 = Decimal String To Number(string=w880, default (0L)=-1 ("default (0 I32)")) -> (number=w883:i32)  [unwired: 1 in, 1 out]
        n552 = in-place {
          in-place-border: w883 -> [w892]
          n553 = in-place-cluster #11(w887) -> ("Control Rules"=w891:T18[])
          n554 = in-place {
            n555 = in-place-array #12(w891, w892) -> (w906:T18)
            n556 = call <vilib>:"Trim Whitespace.vi"("string"="CtrlRule_CustomName") -> ("trimmed string"=w893:string)  [unwired: 1 in]
            n557 = call <vilib>:"Trim Whitespace.vi"("string"="CtrlRule_CtrlID") -> ("trimmed string"=w895:string)  [unwired: 1 in]
            n558 = Empty String/Path?(string/path=w895) -> (empty?=w899:bool)
            n559 = Select(t="<Control ID>", s=w899, f=w895) -> (s? t:f=w896:string)
            n560 = Bundle By Name(cluster=w906, "CtrlID"=w896, "CustomRule"="CtrlRule_CustomRule", "DscrMode"="CtrlRule_DscrMode", "Description"="CtrlRule_Description", "ClusterMembers"="CtrlRule_ClustMembers", "EnumValues"="CtrlRule_EnumValues", "CustomName"=w893) -> (w905:T18)
            n561 = in-place-array #12(w905) -> (w890:T18[])  [unwired: 1 out]
          }
          n562 = in-place-cluster #11("Control Rules"=w890) -> (w886:T15)
        }
        n563 = Concatenate Strings("Globals = Set;\n\nUpdate: Control Rules;\nCtrlRule: Update Controls;" ("string"), w889) -> (w882:string)
        n564 = Bundle(cluster=w885, "Rule out"=w886) -> (w884:cluster{"Array out":string[], "Rule out":T15})  [unwired: 1 in]
      }
      frame "CtrlRule: Enable" {
        n565 = Unbundle(w920) -> ("Rule out"=w922:T15)  [unwired: 1 out]
        n566 = Match Pattern(string=w909, regular expression="\\?") -> (before substring=w915:string, after substring=w913:string)  [unwired: 1 in, 2 out]
        n567 = Decimal String To Number(string=w915) -> (number=w912:i32)  [unwired: 2 in, 1 out]
        n568 = call "VIH Utility - STR - String to 1D Str Array.vi"("delimiter ('\\n')"="," ("delimiter ('\\n')"), "String in"=w913) -> ("Array out"=w911:string[])  [unwired: 5 in]
        n569 = Not Equal To 0?(x=w912) -> (x != 0?=w907:bool)
        n570 = Decimal String To Number(string=w911, default (0L)=-1 ("default (0 I32)")) -> (number=w908:i32[])  [unwired: 1 in, 1 out]
        n571 = in-place {
          in-place-border: w908 -> [w925]
          in-place-border: w907 -> [w924]
          n572 = in-place-cluster #13(w922) -> ("Control Rules"=w927:T18[])
          n573 = for {
            tunnel: w925 -> [w931] mode=indexing
            shift-right: [w929] -> w926
            shift-left: w927 -> [w930]
            tunnel: w924 -> [w928]
            n574 = in-place {
              in-place-border: w928 -> [w932]
              n575 = in-place-array #14(w930, w931) -> (w934:T18)
              n576 = Bundle By Name(cluster=w934, "CustomRule"=w932) -> (w933:T18)
              n577 = in-place-array #14(w933) -> (w929:T18[])  [unwired: 1 out]
            }
          }
          n578 = in-place-cluster #13("Control Rules"=w926) -> (w921:T15)
        }
        n579 = Concatenate Strings("Globals = Set;\n\nUpdate: Control Rules;\nCtrlRule: Update Controls;" ("string"), w923) -> (w918:string)
        n580 = Bundle(cluster=w920, "Rule out"=w921) -> (w919:cluster{"Array out":string[], "Rule out":T15})  [unwired: 1 in]
      }
      frame "CtrlRule: Edit Enum Values" {
        n581 = Unbundle(w941) -> ("Rule out"=w943:T15)  [unwired: 1 out]
        n582 = Decimal String To Number(string=w936, default (0L)=-1 ("default (0 I32)")) -> (number=w939:i32)  [unwired: 1 in, 1 out]
        n583 = in-place {
          in-place-border: w939 -> [w949]
          in-place-border: w935 -> [w946]
          n584 = in-place-cluster #15(w943) -> ("Control Rules"=w948:T18[])
          n585 = in-place {
            in-place-border: w946 -> [w951]
            n586 = in-place-array #16(w948, w949) -> (w955:T18)
            n587 = Unbundle By Name(w955) -> ("EnumValDscr"=w953:T19[], "CtrlID"=w950:string)
            n588 = call "VIH Dialog - Enum Values.vi"("Control ID"=w950, "EnumValDefs in"=w953, "Project Tree"=w951) -> ("OK out"=w954:bool, "EnumValDefs out"=w952:T19[])  [unwired: 7 in]
            n589 = case shown="True" w954 {
              tunnel: [w957 w960] -> w956
              tunnel: w955 -> [w957 w959]
              tunnel: w952 -> [_ w958]
              frame False {
              }
              frame True {
                n590 = Bundle By Name(cluster=w959, "EnumValDscr"=w958) -> (w960:T18)
              }
            }
            n591 = in-place-array #16(w956) -> (w947:T18[])  [unwired: 1 out]
          }
          n592 = in-place-cluster #15("Control Rules"=w947) -> (w942:T15)
        }
        n593 = Concatenate Strings("Globals = Set;\n\nUpdate: Control Rules;\nCtrlRule: Update Controls;" ("string"), w945) -> (w938:string)
        n594 = Bundle(cluster=w941, "Rule out"=w942) -> (w940:cluster{"Array out":string[], "Rule out":T15})  [unwired: 1 in]
      }
      frame "------------------------------ 5" {
      }
      frame "CSS List: Update Controls" {
        n595 = Unbundle(w968) -> ("Rule out"=w967:T15)  [unwired: 1 out]
        n596 = Unbundle By Name(w967) -> ("Source Paths.CSS Files"=w966:path[])
        n597 = Index Array(array=w965) -> (element=w964:i32)  [unwired: 1 in]
        n598 = Empty Array?(array=w965) -> (empty?=w970:bool)
        n599 = call "VIH Utility - UI - Boolean to Control Disable Status.vi"("Status in"=w970) -> ("Control Disable if True"=w969:u8)  [unwired: 3 in, 1 out]
        n600 = Index Array(array=w966, index=w964) -> (element=→"CSS File":path)
        n601 = property on="%CSS List_Remove" class="Bool"("DisabledEnum"=w969) -> ()  [unwired: 2 in, 2 out]
      }
      frame "CSS List: Make Selection Visible" {
        n602 = control-ref of="CSS List"() -> (w978:refnum<vi>)
        n603 = property class="MCListbox (strict)"(reference=w978) -> (reference out=w977:refnum<vi>, "Value"=w976:i32[])  [unwired: 1 in, 1 out]
        n604 = Empty Array?(array=w976) -> (empty?=w975:bool)
        n605 = Index Array(array=w976) -> (element=w974:i32)  [unwired: 1 in]
        n606 = Select(t=-1, s=w975, f=w974) -> (s? t:f=w972:i32)
        n607 = call "VIH Utility - UI - Make Row Visible (MC Listbox).vi"("Row"=w972, "MC Listbox Refnum"=w977) -> ()  [unwired: 8 in, 2 out]
      }
      frame "CSS List: Add" {
        n608 = Array Size(array=w984) -> (size(s)=w982:i32)
        n609 = Unbundle(w994) -> ("Rule out"=w987:T15)  [unwired: 1 out]
        n610 = Unbundle By Name(w987) -> ()  [unwired: 1 out]
        n611 = Array Max & Min(array=w984) -> (max value=w986:i32)  [unwired: 3 out]
        n612 = Less Or Equal To 0?(x=w982) -> (x <= 0?=w983:bool)
        n613 = Select(t=-1, s=w983, f=w986) -> (s? t:f=w985:i32)
        n614 = call "File Dialog"("pattern (all files)"="*.css") -> ("selected paths"=w990:path[], "error out"=w991:errorcluster)  [unwired: 11 in, 2 out]
        n615 = case shown="No Error" w991 {
          tunnel: w987 -> [w1001 w1015]
          tunnel: [w1000 w1015] -> w995
          tunnel: w985 -> [w999 _]
          tunnel: w990 -> [w998 _]
          tunnel: ["Globals = Set;\n\nUpdate: CSS List;\nCSS List: Make Selection Visible;\nCSS List: Update Controls;" ("string") _] -> w988
          frame No Error {
            n616 = in-place {
              in-place-border: w999 -> [w1007]
              in-place-border: w998 -> [w1002]
              n617 = in-place-cluster #17(w1001) -> ("Source Paths.CSS Files"=w1008:path[])
              n618 = Increment(x=w1007) -> (x+1=w1006:i32)
              n619 = Array Size(array=w1008) -> (size(s)=w1009:i32)
              n620 = In Range and Coerce(upper limit=w1009, x=w1006, lower limit=0) -> (coerced(x)=w1005:i32)  [unwired: 1 out]
              n621 = Array Size(array=w1002) -> (size(s)=w1003:i32)
              n622 = for {
                N: w1003 -> [_]
                tunnel: w1005 -> [w1013]
                tunnel: [w1012] -> w1004 mode=indexing
                i -> [w1014]
                n623 = Add(x=w1013, y=w1014) -> (x+y=w1012:i32)
              }
              n624 = Insert Into Array(array=w1008, index=w1005, new element=w1002) -> (w1011:path[])
              n625 = in-place-cluster #17("Source Paths.CSS Files"=w1011) -> (w1000:T15)
              n626 = local write "CSS List"(w1004) -> ()
            }
          }
          frame Error {
          }
        }
        n627 = Concatenate Strings(w988, w996) -> (w992:string)
        n628 = Bundle(cluster=w994, "Rule out"=w995) -> (w993:cluster{"Array out":string[], "Rule out":T15})  [unwired: 1 in]
      }
      frame "CSS List: Remove" {
        n629 = Unbundle(w1020) -> ("Rule out"=w1022:T15)  [unwired: 1 out]
        n630 = in-place {
          in-place-border: w1016 -> [w1036]
          n631 = in-place-cluster #18(w1022) -> ("Source Paths.CSS Files"=w1037:path[])
          n632 = Sort 1D Array(array=w1036) -> (sorted array=w1026:i32[])
          n633 = Reverse 1D Array(array=w1026) -> (reversed array=w1035:i32[])
          n634 = for {
            tunnel: w1035 -> [w1038] mode=indexing
            shift-right: [w1040] -> w1025
            shift-left: w1037 -> [w1039]
            n635 = Delete From Array(array=w1039, index=w1038) -> (array with subset deleted=w1040:path[])  [unwired: 1 in, 1 out]
          }
          n636 = Index Array(array=w1026) -> (element=w1034:i32)  [unwired: 1 in]
          n637 = Array Size(array=w1025) -> (size(s)=w1032:i32)
          n638 = Decrement(x=w1032) -> (x-1=w1027:i32)
          n639 = In Range and Coerce(upper limit=w1027, x=w1034, lower limit=0) -> (coerced(x)=w1030:i32)  [unwired: 1 out]
          n640 = Less Than 0?(x=w1027) -> (x < 0?=w1031:bool)
          n641 = Build Array(w1030) -> (w1029:i32[])
          n642 = in-place-cluster #18("Source Paths.CSS Files"=w1025) -> (w1021:T15)
          n643 = Select(t=i32[] [] ("CSS List"), s=w1031, f=w1029) -> (s? t:f=w1024:i32[])
          n644 = local write "CSS List"(w1024) -> ()
        }
        n645 = Concatenate Strings("Globals = Set;\n\nUpdate: CSS List;\nCSS List: Make Selection Visible;\nCSS List: Update Controls;" ("string"), w1023) -> (w1018:string)
        n646 = Bundle(cluster=w1020, "Rule out"=w1021) -> (w1019:cluster{"Array out":string[], "Rule out":T15})  [unwired: 1 in]
      }
      frame "CSS List: Dragged" {
        n647 = Unbundle(w1044) -> ("Rule out"=w1046:T15)  [unwired: 1 out]
        n648 = in-place {
          n649 = in-place-cluster #19(w1046) -> ("Source Paths.CSS Files"=w1049:path[])
          n650 = property on="CSS List" class="MCListbox (strict)"() -> ("ItemSyms"=w1052:i32[])  [unwired: 2 in, 2 out]
          n651 = call "VIH Utility - UI - Drag and Drop Supporter (w Symbol Indices).vi"("Cmd"=enum16{"make symbols", "test D'n'D"}."test D'n'D", "Item Symbols"=w1052) -> ("indices"=w1050:i32[])  [unwired: 7 in, 2 out]
          n652 = for {
            tunnel: w1050 -> [w1055] mode=indexing
            tunnel: w1049 -> [w1054]
            tunnel: [w1053] -> w1048 mode=indexing
            n653 = Index Array(array=w1054, index=w1055) -> (element=w1053:path)
          }
          n654 = in-place-cluster #19("Source Paths.CSS Files"=w1048) -> (w1045:T15)
        }
        n655 = Concatenate Strings("Globals = Set;\n\nUpdate: CSS List;\n\nCSS List: Update Controls;" ("string"), w1047) -> (w1042:string)
        n656 = Bundle(cluster=w1044, "Rule out"=w1045) -> (w1043:cluster{"Array out":string[], "Rule out":T15})  [unwired: 1 in]
      }
      frame "------------------------------ 6" {
      }
      frame "JS List: Update Controls" {
        n657 = Unbundle(w1063) -> ("Rule out"=w1062:T15)  [unwired: 1 out]
        n658 = Unbundle By Name(w1062) -> ("Source Paths.JS Files"=w1061:path[])
        n659 = Index Array(array=w1058) -> (element=w1060:i32)  [unwired: 1 in]
        n660 = Empty Array?(array=w1058) -> (empty?=w1065:bool)
        n661 = call "VIH Utility - UI - Boolean to Control Disable Status.vi"("Status in"=w1065) -> ("Control Disable if True"=w1064:u8)  [unwired: 3 in, 1 out]
        n662 = Index Array(array=w1061, index=w1060) -> (element=→"JS File":path)
        n663 = property on="%JS List_Remove" class="Bool"("DisabledEnum"=w1064) -> ()  [unwired: 2 in, 2 out]
      }
      frame "JS List: Make Selection Visible" {
        n664 = control-ref of="JS List"() -> (w1073:refnum<vi>)
        n665 = property class="MCListbox (strict)"(reference=w1073) -> (reference out=w1072:refnum<vi>, "Value"=w1071:i32[])  [unwired: 1 in, 1 out]
        n666 = Empty Array?(array=w1071) -> (empty?=w1070:bool)
        n667 = Index Array(array=w1071) -> (element=w1069:i32)  [unwired: 1 in]
        n668 = Select(t=-1, s=w1070, f=w1069) -> (s? t:f=w1067:i32)
        n669 = call "VIH Utility - UI - Make Row Visible (MC Listbox).vi"("Row"=w1067, "MC Listbox Refnum"=w1072) -> ()  [unwired: 8 in, 2 out]
      }
      frame "JS List: Add" {
        n670 = Array Size(array=w1077) -> (size(s)=w1079:i32)
        n671 = Unbundle(w1089) -> ("Rule out"=w1082:T15)  [unwired: 1 out]
        n672 = Unbundle By Name(w1082) -> ()  [unwired: 1 out]
        n673 = Array Max & Min(array=w1077) -> (max value=w1081:i32)  [unwired: 3 out]
        n674 = Less Or Equal To 0?(x=w1079) -> (x <= 0?=w1080:bool)
        n675 = Select(t=-1, s=w1080, f=w1081) -> (s? t:f=w1078:i32)
        n676 = call "File Dialog2"("pattern (all files)"="*.js") -> ("selected paths"=w1085:path[], "error out"=w1086:errorcluster)  [unwired: 11 in, 2 out]
        n677 = case shown="No Error" w1086 {
          tunnel: w1082 -> [w1096 w1110]
          tunnel: [w1095 w1110] -> w1090
          tunnel: w1078 -> [w1094 _]
          tunnel: w1085 -> [w1093 _]
          tunnel: ["Globals = Set;\n\nUpdate: JS List;\nJS List: Make Selection Visible;\nJS List: Update Controls;" ("string") _] -> w1083
          frame No Error {
            n678 = in-place {
              in-place-border: w1094 -> [w1102]
              in-place-border: w1093 -> [w1097]
              n679 = in-place-cluster #20(w1096) -> ("Source Paths.JS Files"=w1103:path[])
              n680 = Increment(x=w1102) -> (x+1=w1101:i32)
              n681 = Array Size(array=w1103) -> (size(s)=w1104:i32)
              n682 = In Range and Coerce(upper limit=w1104, x=w1101, lower limit=0) -> (coerced(x)=w1100:i32)  [unwired: 1 out]
              n683 = Array Size(array=w1097) -> (size(s)=w1098:i32)
              n684 = for {
                N: w1098 -> [_]
                tunnel: w1100 -> [w1108]
                tunnel: [w1107] -> w1099 mode=indexing
                i -> [w1109]
                n685 = Add(x=w1108, y=w1109) -> (x+y=w1107:i32)
              }
              n686 = Insert Into Array(array=w1103, index=w1100, new element=w1097) -> (w1106:path[])
              n687 = in-place-cluster #20("Source Paths.JS Files"=w1106) -> (w1095:T15)
              n688 = local write "JS List"(w1099) -> ()
            }
          }
          frame Error {
          }
        }
        n689 = Concatenate Strings(w1083, w1091) -> (w1087:string)
        n690 = Bundle(cluster=w1089, "Rule out"=w1090) -> (w1088:cluster{"Array out":string[], "Rule out":T15})  [unwired: 1 in]
      }
      frame "JS List: Remove" {
        n691 = Unbundle(w1115) -> ("Rule out"=w1117:T15)  [unwired: 1 out]
        n692 = in-place {
          in-place-border: w1111 -> [w1131]
          n693 = in-place-cluster #21(w1117) -> ("Source Paths.JS Files"=w1132:path[])
          n694 = Sort 1D Array(array=w1131) -> (sorted array=w1129:i32[])
          n695 = Reverse 1D Array(array=w1129) -> (reversed array=w1130:i32[])
          n696 = for {
            tunnel: w1130 -> [w1133] mode=indexing
            shift-right: [w1135] -> w1126
            shift-left: w1132 -> [w1134]
            n697 = Delete From Array(array=w1134, index=w1133) -> (array with subset deleted=w1135:path[])  [unwired: 1 in, 1 out]
          }
          n698 = Index Array(array=w1129) -> (element=w1128:i32)  [unwired: 1 in]
          n699 = Array Size(array=w1126) -> (size(s)=w1125:i32)
          n700 = Decrement(x=w1125) -> (x-1=w1119:i32)
          n701 = In Range and Coerce(upper limit=w1119, x=w1128, lower limit=0) -> (coerced(x)=w1123:i32)  [unwired: 1 out]
          n702 = Less Than 0?(x=w1119) -> (x < 0?=w1124:bool)
          n703 = Build Array(w1123) -> (w1122:i32[])
          n704 = Select(t=i32[] [] ("CSS List"), s=w1124, f=w1122) -> (s? t:f=w1120:i32[])
          n705 = in-place-cluster #21("Source Paths.JS Files"=w1126) -> (w1116:T15)
          n706 = local write "JS List"(w1120) -> ()
        }
        n707 = Concatenate Strings("Globals = Set;\n\nUpdate: JS List;\nJS List: Make Selection Visible;\nJS List: Update Controls;" ("string"), w1118) -> (w1113:string)
        n708 = Bundle(cluster=w1115, "Rule out"=w1116) -> (w1114:cluster{"Array out":string[], "Rule out":T15})  [unwired: 1 in]
      }
      frame "JS List: Dragged" {
        n709 = Unbundle(w1139) -> ("Rule out"=w1141:T15)  [unwired: 1 out]
        n710 = in-place {
          n711 = in-place-cluster #22(w1141) -> ("Source Paths.JS Files"=w1144:path[])
          n712 = property on="JS List" class="MCListbox (strict)"() -> ("ItemSyms"=w1147:i32[])  [unwired: 2 in, 2 out]
          n713 = call "VIH Utility - UI - Drag and Drop Supporter (w Symbol Indices).vi"("Cmd"=enum16{"make symbols", "test D'n'D"}."test D'n'D", "Item Symbols"=w1147) -> ("indices"=w1145:i32[])  [unwired: 7 in, 2 out]
          n714 = for {
            tunnel: w1145 -> [w1150] mode=indexing
            tunnel: w1144 -> [w1149]
            tunnel: [w1148] -> w1143 mode=indexing
            n715 = Index Array(array=w1149, index=w1150) -> (element=w1148:path)
          }
          n716 = in-place-cluster #22("Source Paths.JS Files"=w1143) -> (w1140:T15)
        }
        n717 = Concatenate Strings("Globals = Set;\n\nUpdate: JS List;\n\nJS List: Update Controls;" ("string"), w1142) -> (w1137:string)
        n718 = Bundle(cluster=w1139, "Rule out"=w1140) -> (w1138:cluster{"Array out":string[], "Rule out":T15})  [unwired: 1 in]
      }
      frame "------------------------------ 7" {
      }
    }
  }
  n719 = while {
    shift-right: [w1157] -> _
    shift-left: "INIT;" -> [w1160]
    tunnel: w2 -> [w1154]
    tunnel: w3 -> [w1153]
    stop <- w1155 stop-if-true
    n720 = call "VIH Utility - APP - State Queue Parser (STR).vi"("input queue"=w1160) -> ("state"=w1159:string, "remained queue"=w1156:string, "complete state specifier"=w1158:string)  [unwired: 5 in, 1 out]
    n721 = case shown="\"\"" w1159 {
      tunnel: w1158 -> [w1166 _ _ _]
      tunnel: [w1161 w1171 w1173 w1181] -> w1157
      tunnel: w1156 -> [w1162 w1171 w1173 w1180]
      tunnel: [_ _ TRUE _] -> w1155
      tunnel: w1154 -> [_ _ w1172 w1184]
      tunnel: w1153 -> [_ _ _ w1179]
      frame Default {
        n722 = property class="VI"() -> ("Name"=w1165:string)  [unwired: 2 in, 2 out]
        n723 = Format Into String(format string="%s\n(Communication Loop)\n\nUnknown state specifier:\n%s", w1165, w1166) -> (resulting string=w1169:string)  [unwired: 2 in, 1 out]
        n724 = Two Button Dialog(message=w1169, 1:"HALT" ("F button name (\"Cancel\")"), 2:"Continue" ("T button name (\"OK\")")) -> (T button?=w1163:bool)
        n725 = Select(t=w1162, s=w1163, f="HALT;") -> (s? t:f=w1161:string)
      }
      frame "INIT" {
      }
      frame "HALT" {
        n726 = Release Queue(queue=w1172) -> ()  [unwired: 2 in, 3 out]
      }
      frame "" {
        n727 = Dequeue Element(queue=w1184, timeout in ms (-1)=200) -> (element=w1175:T8, error out=w1183:errorcluster)  [unwired: 1 in, 2 out]
        n728 = Unbundle By Name(w1175) -> ("Action"=w1177:string)
        n729 = Empty String/Path?(string/path=w1177) -> (empty?=w1176:bool)
        n730 = case shown="False" w1176 {
          tunnel: w1179 -> [w1186 _]
          tunnel: w1175 -> [w1185 _]
          frame False {
            n731 = Generate User Event(user event=w1186, event data cluster=w1185) -> ()  [unwired: 2 in, 2 out]
          }
          frame True {
          }
        }
        n732 = Select(t="HALT;", s=w1183, f=w1180) -> (s? t:f=w1181:string)
      }
    }
  }
